vi "AFM_Lithography.vi"() -> ()   [LabVIEW 2019]
uses:
  subVIs/Global Variables.vi
  <vilib>/Analysis/Matrix/Datatypes/RealMatrix.ctl
  <vilib>/Analysis/Matrix/NI_Matrix.lvlib
  <userlib>/LevyLab/Relay Box/Typedefs/Resistor--enum.ctl
  <userlib>/LevyLab/Relay Box/Relay-Box.lvclass
  subVIs/AFM API/AFM_Driver_Manager/AFM_Driver_Manager.lvclass
  <vilib>/vision/Image Controls.llb/IMAQ Image.ctl
  <userlib>/LevyLab/Configuration/Configuration.lvclass
  Controls/Configuration.ctl
  Classes/Parse/ParseVectorFile/ParseVectorFile.lvclass
  <vilib>/JKI/JKI SMO/SMO/SMO.lvclass
  Classes/Settings/Setting Database/Setting Database.lvclass
  Classes/Settings/Setting Database/Typedefs/PrivateEvents--Setting Database.Refresh.ctl
  Classes/Parse/Dot/Dot.lvclass
  Classes/Settings/Dot Settings/Dot Settings.lvclass
  Classes/Settings/Path Settings/Path Settings.lvclass
  Classes/Tool/Tool Data/Tool Data/Tool Data.lvclass
  Classes/Settings/Setting Database/Typedefs/PublicEvents--Setting Database.PathsUpdated.ctl
  Classes/Settings/Rectangle Settings/Rectangle Settings.lvclass
  Classes/Settings/Setting Database/Typedefs/PublicEvents--Setting Database.RectanglesUpdated.ctl
  Classes/Settings/Funnel Settings/Funnel Settings.lvclass
  Classes/Settings/Setting Database/Typedefs/PublicEvents--Setting Database.FunnelsUpdated.ctl
  Classes/Settings/Setting Database/Typedefs/PublicEvents--Setting Database.DotsUpdated.ctl
  Classes/Parse/ParsePaths/Path.lvclass
  Classes/Parse/Rectangle/Rectangle.lvclass
  Classes/Parse/Image/SVGImage.lvclass
  Classes/Tool/Tool Data/Tool Data/Typedefs/PrivateEvents--Tool Data.Update Objects.ctl
  <vilib>/Platform/browser.llb/Open URL in Default Browser (string).vi
  Classes/Selector/Selector.lvclass
  <vilib>/Utility/miscctls.llb/LVPositionTypeDef.ctl
  Classes/Settings/ObjectSettings/ObjectSettings.lvclass
  C:/Program Files (x86)/National Instruments/LabVIEW 2019/vi.lib/JKI/JKI SMO/SMO/SMO.lvclass
  C:/Users/Albro/Documents/GitHub/AFM-Lithography/lvsrc/Classes/Settings/ObjectSettings/ObjectSettings.lvclass
  Classes/Tool/Tool Path/Tool Path.lvclass
  Classes/Tool/Tool Funnel/Tool Funnel.lvclass
  Classes/Tool/Tool Rectangle/Tool Rectangle.lvclass
  Classes/Tool/Tool Dot/Tool Dots.lvclass
panel:
  in  "Listbox":i32(listbox)
  out "version":string
  out "Ready?":bool
  out "Estimated Time":string
  in  "Run":bool
  in  "Refresh Button":bool
  in  "Done":bool
  in  "Help":bool
  in  "Abort":bool
  out "Render":T1(plugin-control)
  in  "Settings":T2(tab)
  out "Status":string
  in  "Background Image":path caption="Path"
  in  "Inkscape File (.svg)":path caption="Path"
  in  "Hide Labels?":bool
  in  "Patterns":i32(listbox) caption="Patterns (drag-and-drop reorder)"
  in  "AFM Type":u16(ring) caption="Ring" items=["Asylum"]
  in  "Save Render":bool caption="Save"
  in  "Autosave?":bool
  in  "Autosave Path":path caption="Path"
  in  "Create Overlay":bool
  out "Image Filename":string
  in  "Image Data Range":cluster{dbl, dbl}(slide)={100.0, 0.0} scale=0.0..100.0
  in  "Page":u32 caption="Numeric" max=3
  in  "MCLB":i32(listbox) caption="Multicolumn Listbox 2"
  # "AFM Lithography"
  # "Render"
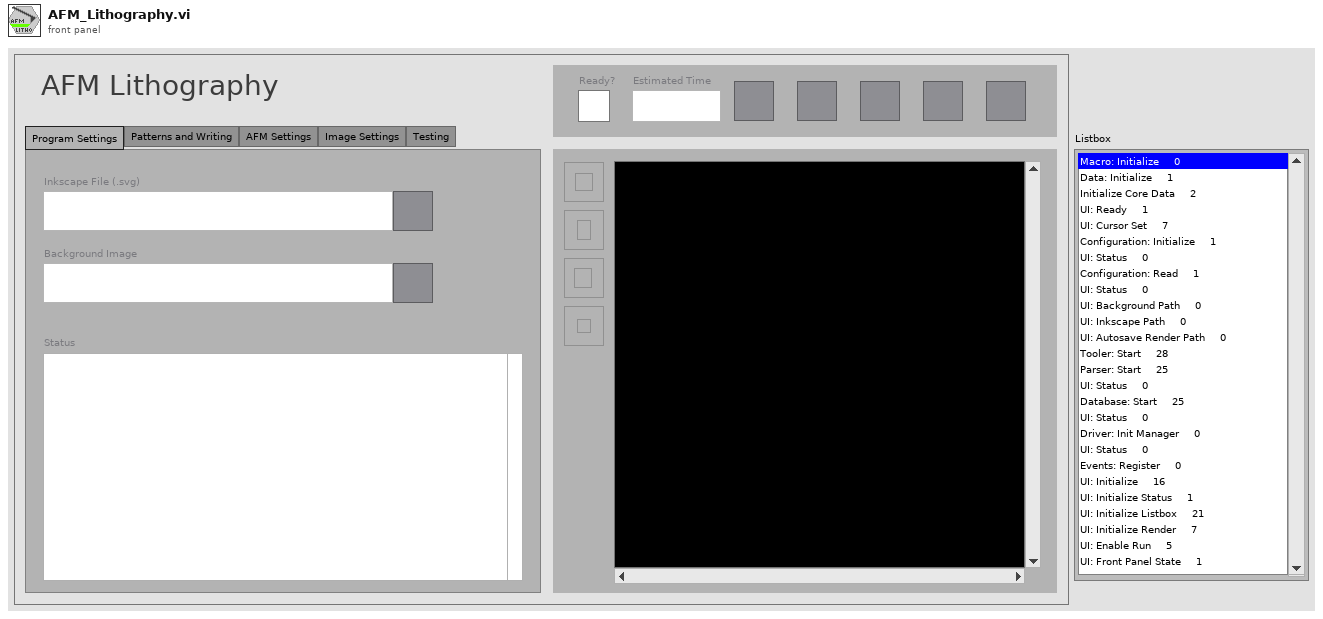
[diagram p1: front panel]
types:
  T1 = typedef "IMAQ Image.ctl" = refnum<image>
  T2 = enum32{"Program Settings", "Patterns and Writing", "AFM Settings", "Image Settings", "Testing"}
  T3 = typedef "LVPositionTypeDef.ctl" = cluster{"Left":i32, "Top":i32}
  T4 = cluster{"Point":T3, "Button":u16, "PlatMods":cluster{"Shift":bool, "Ctrl":bool, "Alt":bool, "Cmd":bool, "Opt":bool}}
  T5 = enum32{"invalid app kind", "Development System", "Run Time System", "Student Edition", "Embedded LabVIEW", "Evaluation", "Custom"}
  T6 = enum32{"Program Settings", "Patterns and Writing", "AFM Settings", "Image Settings"}
  T7 = enum32{"Invalid", "Standard", "Closed", "Hidden", "Minimized", "Maximized"}
  T8 = enum8{"Enabled", "Disabled", "Disabled and Grayed Out"}
  T9 = cluster{"Pattern":string, "Pattern Label":string, "Prompt":string}
  T10 = cluster{"Name":string, "Group":string, "Enabled":bool}
  T11 = typedef "Configuration.ctl" = cluster{"Inkscape Path":path, "Background Path":path, "Autosave Render Path":path, "Autosave Render":bool, "Hide Labels":bool, "Normal Render Path":path, "Overwrite":bool}
  T12 = typedef "Setting Database.lvclass/PrivateEvents--Setting Database.Refresh.ctl" = cluster{"Paths":string[], "Rectangles":string[], "Funnels":string[], "Dots":string[]}
  T13 = typedef "Tool Data.lvclass/PrivateEvents--Tool Data.Update Objects.ctl" = cluster{"Settings":cluster{"Paths":T14, "Rectangles":T15, "Funnels":T16, "Dots":T17}, "Data":cluster{"Paths":refnum<class "Path.lvclass">[], "Rectangles":refnum<class "Rectangle.lvclass">[], "SVGImage":refnum<class "SVGImage.lvclass">, "Dots":refnum<class "Dot.lvclass">[], "Funnels":refnum<class "Path.lvclass">[]}}
  T14 = typedef "Setting Database.lvclass/PublicEvents--Setting Database.PathsUpdated.ctl" = refnum<class "Path Settings.lvclass">[]
  T15 = typedef "Setting Database.lvclass/PublicEvents--Setting Database.RectanglesUpdated.ctl" = refnum<class "Rectangle Settings.lvclass">[]
  T16 = typedef "Setting Database.lvclass/PublicEvents--Setting Database.FunnelsUpdated.ctl" = refnum<class "Funnel Settings.lvclass">[]
  T17 = typedef "Setting Database.lvclass/PublicEvents--Setting Database.DotsUpdated.ctl" = refnum<class "Dot Settings.lvclass">[]
  T18 = typedef "NI_Matrix.lvlib/RealMatrix.ctl" = dbl[][]
  T19 = typedef "Relay-Box.lvclass/Resistor--enum.ctl" = enum16{"open", "discharge tip", "0 ohms", "100k ohm", "10M ohm", "1G ohm"}
  T20 = cluster{"Core":cluster{"Current VI Reference":refnum<vi>, "Close Panel on Exit?":bool}, "Parsing Data":cluster{"paths":cluster{"Fill Color":string, "Stroke Color":string, "Commands":cluster{"Command Type":string, "Coordinates":cluster{"X":dbl, "Y":dbl}[]}[], "Transformation Matrix 2":T18}[], "funnels":cluster{"Fill Color":string, "Stroke Color":string, "Commands":cluster{"Command Type":string, "Coordinates":cluster{"X":dbl, "Y":dbl}[]}[], "Transformation Matrix 2":T18}[], "rects":cluster{"Fill Color":string, "Stroke Color":string, "Width":dbl, "Height":dbl, "X":dbl, "Y":dbl, "Transformation Matrix":T18}[], "Dots":refnum<class "Dot.lvclass">[]}, "Lithography Data":cluster{"Name":string, "Litho":cluster{"X":dbl, "Y":dbl, "Speed":dbl, "Voltage":dbl}[], "Set Resistance":T19, "Meta":variant}[], "VI Refs":refnum<vi>[], "root path":path, "AFM_Driver_Manager":refnum<class "AFM_Driver_Manager.lvclass">, "IMAQ (Work)":T1, "Background Image":path, "Inkscape File (.svg)":path, "ParseVectorFile":refnum<class "ParseVectorFile.lvclass">, "Database":refnum<class "Setting Database.lvclass">, "Hide Labels":bool, "Autosave?":bool, "Autosave Path":path, "Image Data Range":cluster{dbl, dbl}, "Status":string, "Config":refnum<class "Configuration.lvclass">, "Drag and Drop":cluster{"Start":string[], "End":string[], "Running":string[], "Working":string[]}, "IDs":cluster{"paths":string[], "funnels":string[], "rects":string[], "dots":string[]}, "Tooler":refnum<class "Tool Data.lvclass">, "MCLB":refnum<class "Selector.lvclass">, "Menu Path":string, "Item Names":string[][]}
  T21 = cluster{"Paths":T14, "Rectangles":T15, "Funnels":T16, "Dots":T17}
  T22 = typedef "LVPoint32TypeDef.ctl" = cluster{"Horizontal":i32, "Vertical":i32}
  T23 = cluster{"Shift":bool, "Ctrl":bool, "Alt":bool, "Cmd":bool, "Opt":bool}
  T24 = cluster{"paths":string[], "funnels":string[], "rects":string[], "dots":string[]}
  T25 = cluster{"Start":string[], "End":string[], "Running":string[], "Working":string[]}
  T26 = cluster{"paths":cluster{"Fill Color":string, "Stroke Color":string, "Commands":cluster{"Command Type":string, "Coordinates":cluster{"X":dbl, "Y":dbl}[]}[], "Transformation Matrix 2":T18}[], "funnels":cluster{"Fill Color":string, "Stroke Color":string, "Commands":cluster{"Command Type":string, "Coordinates":cluster{"X":dbl, "Y":dbl}[]}[], "Transformation Matrix 2":T18}[], "rects":cluster{"Fill Color":string, "Stroke Color":string, "Width":dbl, "Height":dbl, "X":dbl, "Y":dbl, "Transformation Matrix":T18}[], "Dots":refnum<class "Dot.lvclass">[]}
  T27 = cluster{"Name":string, "Litho":cluster{"X":dbl, "Y":dbl, "Speed":dbl, "Voltage":dbl}[], "Set Resistance":T19, "Meta":variant}[]
  T28 = cluster{"Current VI Reference":refnum<vi>, "Close Panel on Exit?":bool}
  T29 = typedef "Setting Database.lvclass/PublicEvents--Cluster.ctl" = cluster{"NewActivePath":refnum<user-event>, "PathsUpdated":refnum<user-event>, "RectanglesUpdated":refnum<user-event>, "NewActiveRectangle":refnum<user-event>, "NewActiveFunnel":refnum<user-event>, "FunnelsUpdated":refnum<user-event>, "NewActiveDot":refnum<user-event>, "DotsUpdated":refnum<user-event>}
  T30 = typedef "AFM_Driver_Manager.lvclass/AFM_Driver_Manager.PublicEvents.ctl" = cluster{"Lithography Done":refnum<user-event>}
  T31 = typedef "Image Type" = u32
  T32 = cluster{"Name":string, "Litho":cluster{"X":dbl, "Y":dbl, "Speed":dbl, "Voltage":dbl}[], "Set Resistance":T19, "Meta":variant}
  T33 = cluster{"Name":string, "Group":string, "Enabled":bool}[]
  T34 = typedef "ParseVectorFile.lvclass/PublicEvents--ParseVectorFile.ParsedData.ctl" = cluster{"Paths":refnum<class "Path.lvclass">[], "Rectangles":refnum<class "Rectangle.lvclass">[], "Background":refnum<class "SVGImage.lvclass">, "Dots":refnum<class "Dot.lvclass">[], "Other Images":refnum<class "SVGImage.lvclass">[]}
  T35 = cluster{"Paths":refnum<class "Path.lvclass">[], "Rectangles":refnum<class "Rectangle.lvclass">[], "SVGImage":refnum<class "SVGImage.lvclass">, "Dots":refnum<class "Dot.lvclass">[], "Funnels":refnum<class "Path.lvclass">[]}
  T36 = typedef "Tool Data.lvclass/PublicEvents--Tool Data.Objects Updated.ctl" = cluster{"Paths":refnum<class "Tool Path.lvclass">[], "Funnels":refnum<class "Tool Funnel.lvclass">[], "Rectangles":refnum<class "Tool Rectangle.lvclass">[], "Dots":refnum<class "Tool Dots.lvclass">[]}
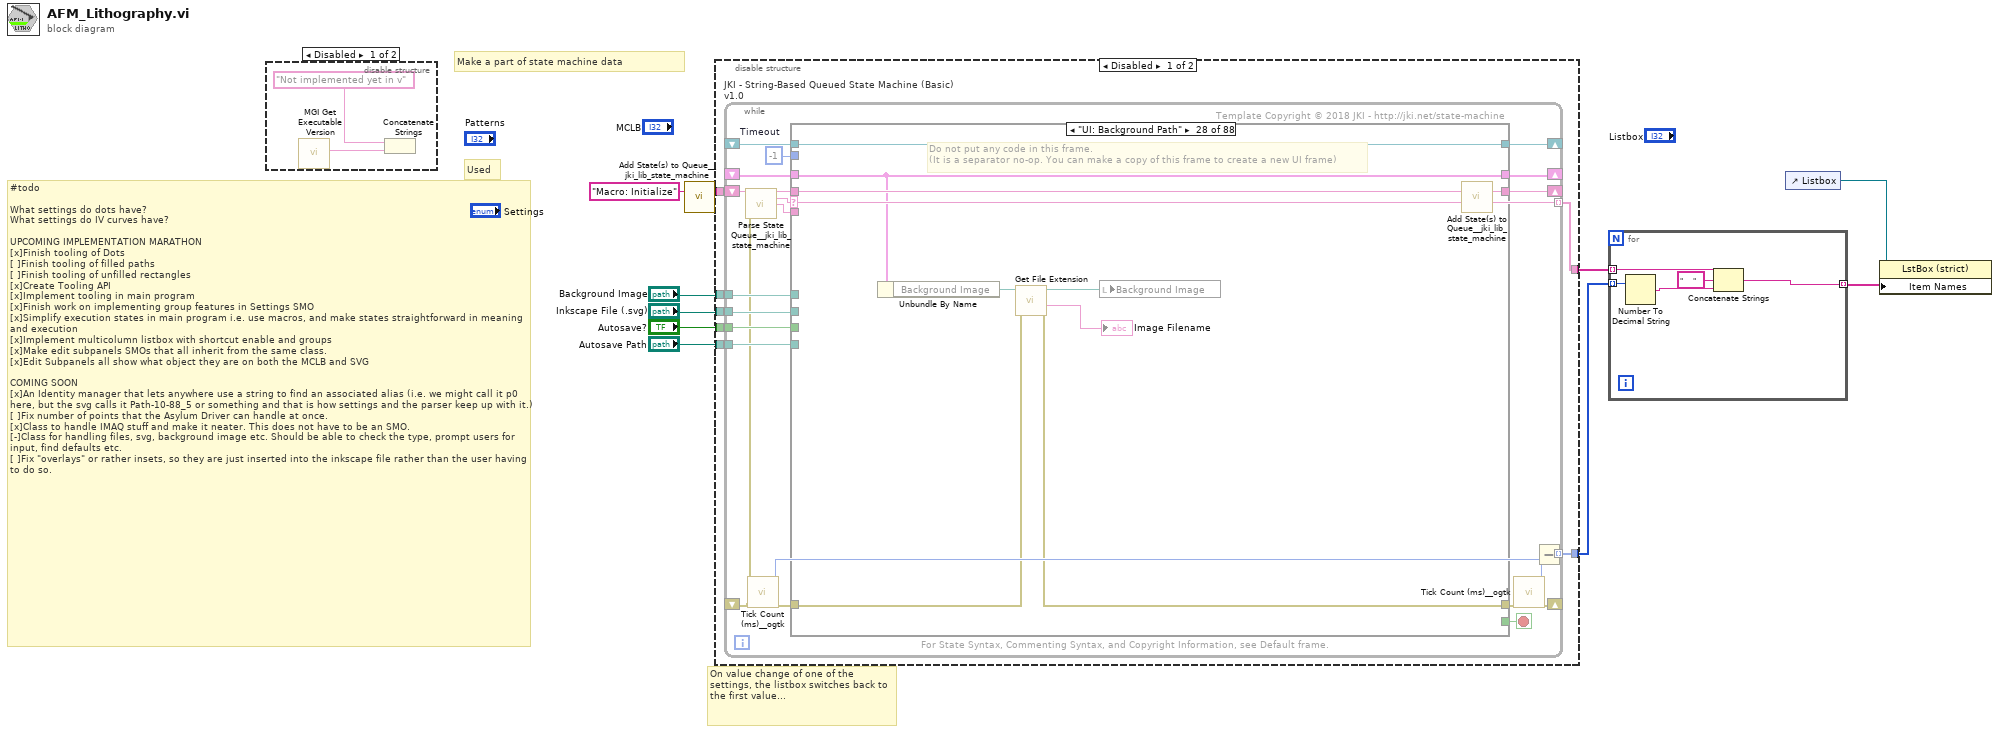
[diagram p0: block diagram]
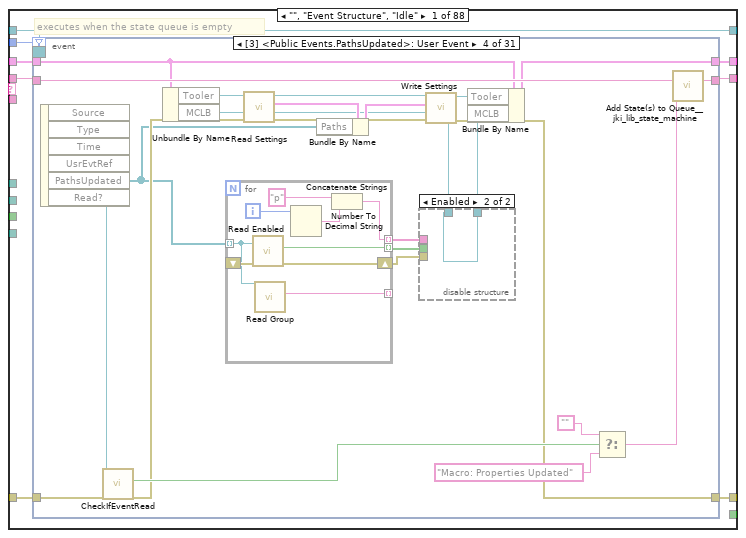
[diagram p2: hidden frame]
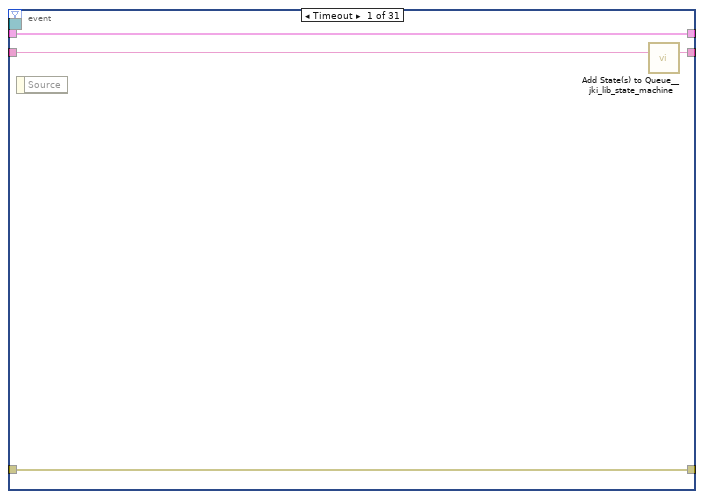
[diagram p3: hidden frame]
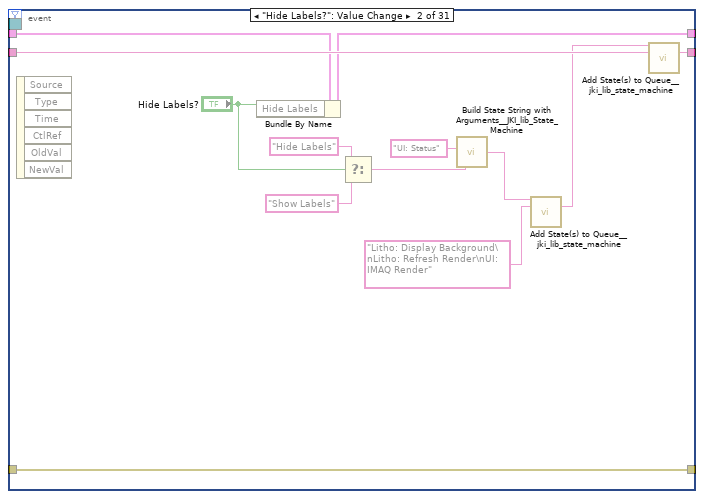
[diagram p4: hidden frame]
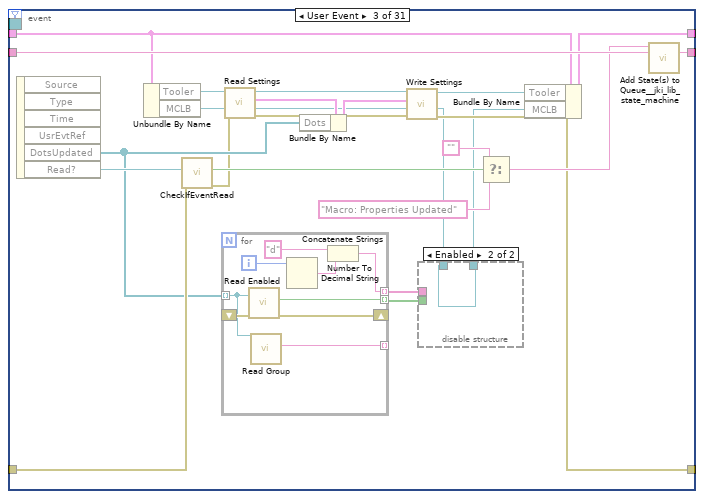
[diagram p5: hidden frame]
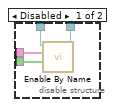
[diagram p6: hidden frame]
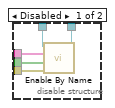
[diagram p7: hidden frame]
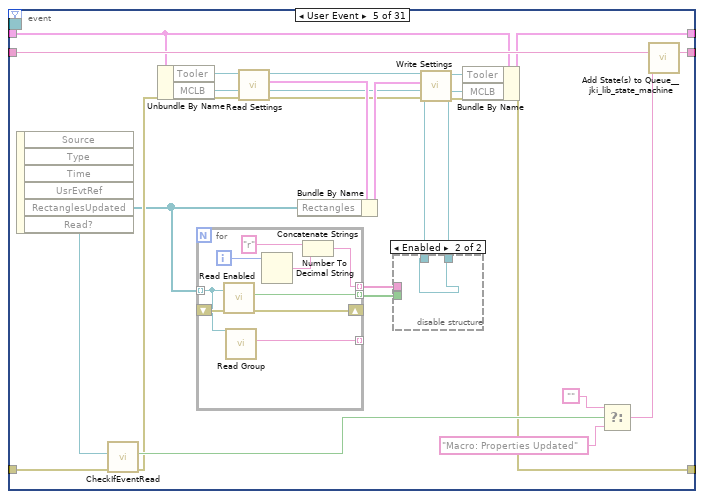
[diagram p8: hidden frame]
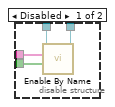
[diagram p9: hidden frame]
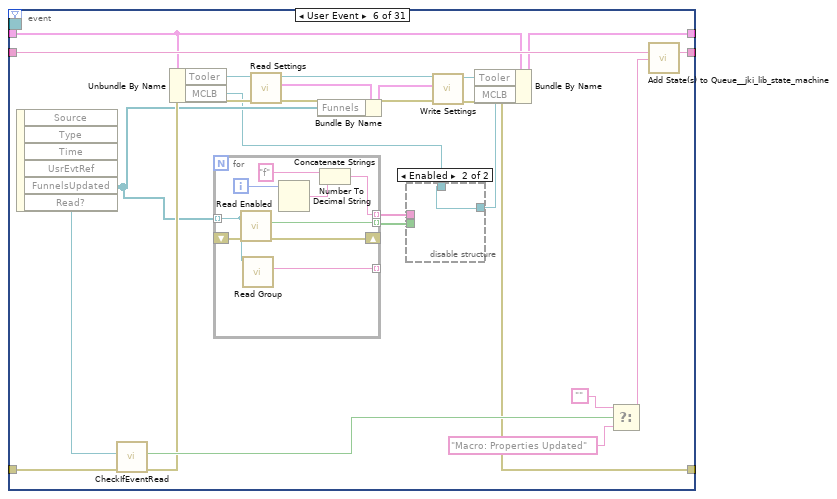
[diagram p10: hidden frame]
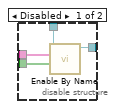
[diagram p11: hidden frame]
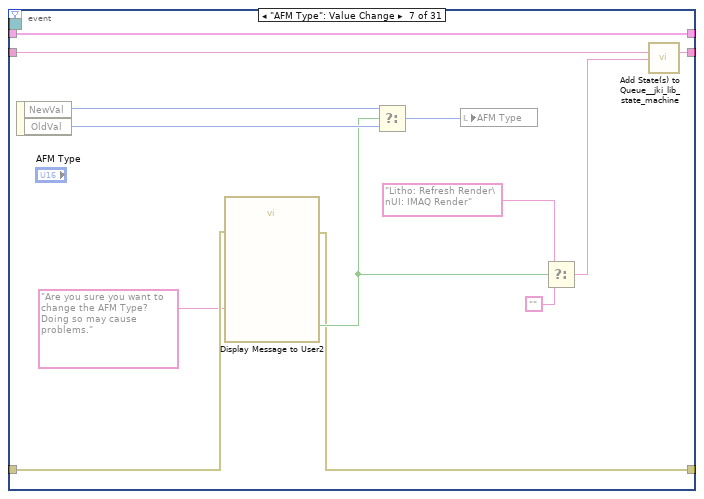
[diagram p12: hidden frame]
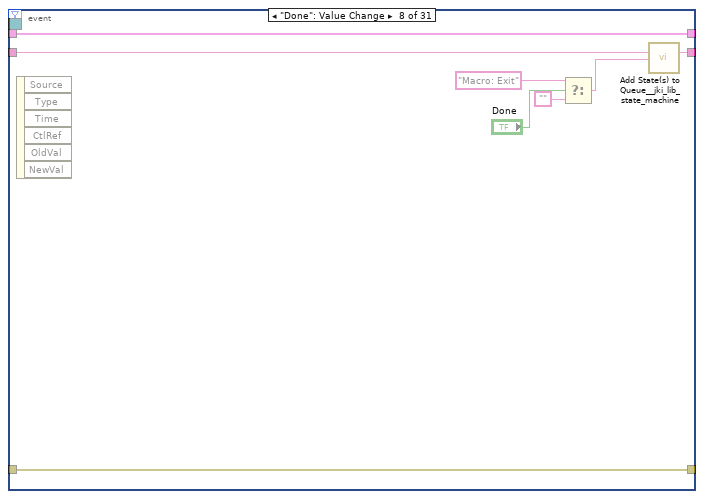
[diagram p13: hidden frame]
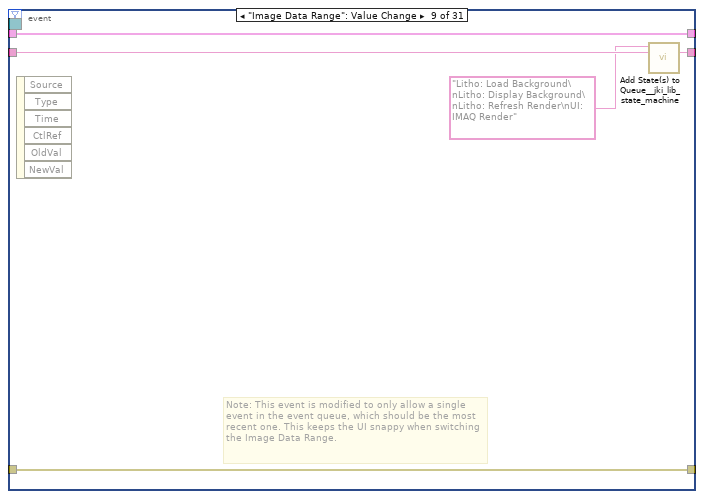
[diagram p14: hidden frame]
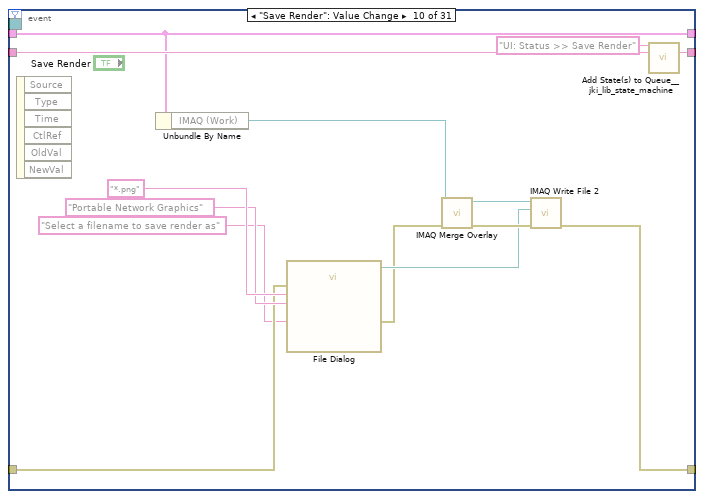
[diagram p15: hidden frame]
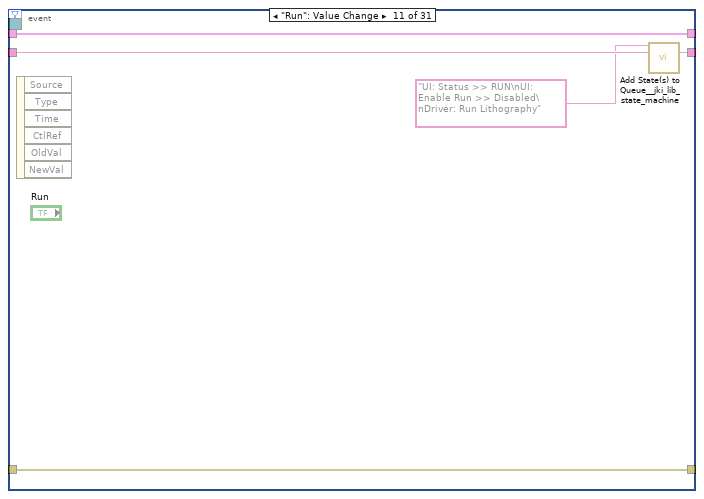
[diagram p16: hidden frame]
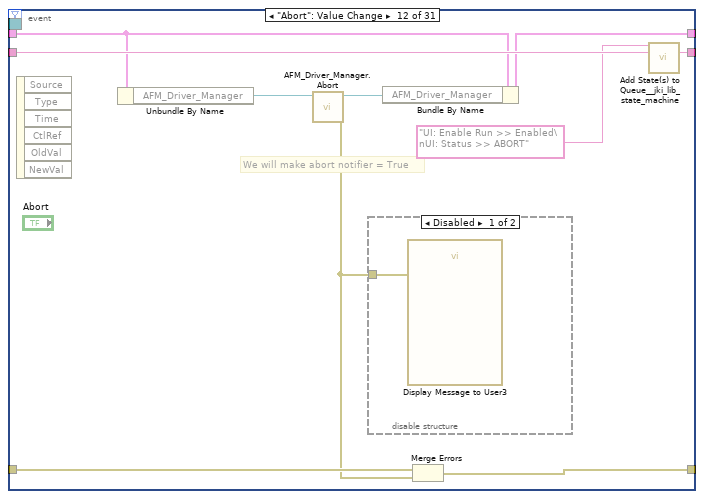
[diagram p17: hidden frame]
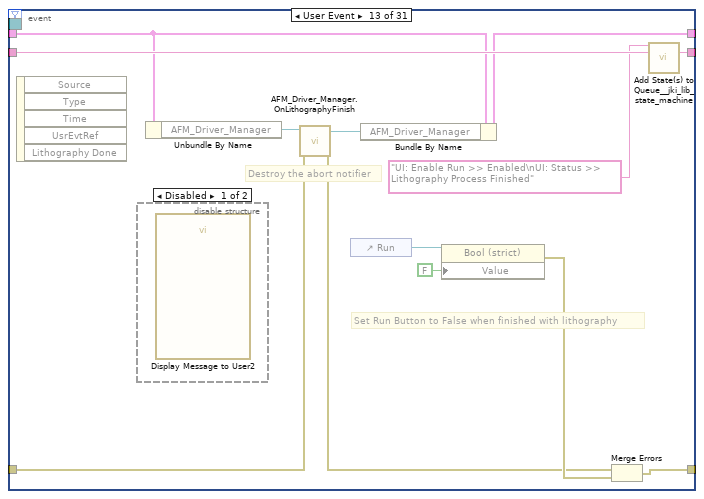
[diagram p19: hidden frame]
diagram:
  # "On value change of one of the settings, the listbox switches back to the first value..."
  # "#todo\n\nWhat settings do dots have?\nWhat settings do IV curves have?\n\nUPCOMING IMPLEMENTATION MARATHON\n[x]Finish tooling of Dots\n[ ]Finish tooling of filled paths\n[ ]Finish tooling of unfilled rectangles\n[x]Create Tooling API\n[x]Implement tooling in main program\n[x]Finish work on implementing group features in Settings SMO\n[x]Simplify execution states in main program i.e. use macros, and make states straightforward in meaning and execution\n[x]Implement multicolumn listbox with shortcut enable and groups\n[x]Make edit subpanels SMOs that all inherit from the same class.\n[x]Edit Subpanels all show what object they are on both the MCLB and SVG\n\nCOMING SOON\n[x]An Identity manager that lets anywhere use a string to find an associated alias (i.e. we might call it p0 here, but the svg calls it Path-10-88_5 or something and that is how settings and the parser keep up with it.)\n[ ]Fix number of points that the Asylum Driver can handle at once.\n[x]Class to handle IMAQ stuff and make it neater. This does not have to be an SMO.\n[-]Class for handling files, svg, background image etc. Should be able to check the type, prompt users for input, find defaults etc.\n[ ]Fix \"overlays\" or rather insets, so they are just inserted into the inkscape file rather than the user having to do so."
  # "Used"
  # "Make a part of state machine data"
  n1 = disable-structure shown="Disabled" {
    frame Disabled {
      n2 = call <userlib>:"MGI Get Executable Version.vi"() -> ("Version"=w11:string)  [unwired: 7 in]
      n3 = Concatenate Strings("Not implemented yet in v" ("Status"), w11) -> ()  [unwired: 1 out]
    }
    frame Enabled {
    }
  }
  n4 = call <vilib>:"Add State(s) to Queue__jki_lib_state_machine.vi"("State(s) in (\"\")"="Macro: Initialize") -> ("States Out"=w10:string)  [unwired: 14 in]
  n5 = disable-structure shown="Disabled" {
    disable-tunnel: w10 -> [w19 _]
    disable-tunnel: "Background Image" -> [w18 _]
    disable-tunnel: "Inkscape File (.svg)" -> [w17 _]
    disable-tunnel: "Autosave?" -> [w16 _]
    disable-tunnel: "Autosave Path" -> [w15 _]
    disable-tunnel: [w14 _] -> w4
    disable-tunnel: [w13 _] -> w3
    frame Disabled {
      n6 = while "JKI - String-Based Queued State Machine (Basic) v1.0" {
        shift-right: [w39] -> _
        shift-left: _ -> [w38]
        shift-right: [w24] -> _
        shift-left: _ -> [w26]
        shift-right: [w29] -> _
        shift-left: w19 -> [w41]
        shift-right: [w35] -> _
        shift-left: _ -> [w34]
        tunnel: w18 -> [w33]
        tunnel: w17 -> [w32]
        tunnel: w16 -> [w31]
        tunnel: w15 -> [w30]
        tunnel: [w25] -> w14 mode=indexing
        tunnel: [w20] -> w13 mode=indexing
        stop <- w40 stop-if-true
        w37 = -1  # Timeout
        # "Template Copyright © 2018 JKI - http://jki.net/state-machine"
        # "For State Syntax, Commenting Syntax, and Copyright Information, see Default frame."
        n7 = call <vilib>:"Parse State Queue__jki_lib_state_machine.vi"("State Queue"=w41, "Error In (no error)"=w26) -> ("Remaining States"=w36:string, "Current State"=w25:string, "Arguments"=w28:string)  [unwired: 11 in]
        n8 = call <userlib>:"Tick Count (ms)__ogtk.vi"("error in (no error)"=w26) -> ("error out"=w23:errorcluster, "millisecond timer value"=w21:u32)  [unwired: 9 in]
        n9 = case shown="\"UI: Background Path\"" w25 {
          selector: w25 -> [_ _ w478 _ _ _ _ _ _ _ _ _ _ _ _ _ _ _ _ _ _ _ _ _ _ _ _ _ _ _ _ _ _ _ _ _ _ _ _ _ _ _ _ _ _ _ _ _ _ _ _ _ _ _ _ _ _ _ _ _ _ _ _ _ _ _ _ _ _ _ _ _ _ _ _ _ _ _ _ _ _ _ _ _ _ _ _ _]
          tunnel: w28 -> [_ _ _ _ w505 _ _ _ _ _ _ _ _ _ _ _ _ _ _ w688 w700 w708 w724 w735 _ w778 _ _ _ _ _ _ _ _ _ _ _ _ _ _ _ _ _ _ _ _ _ _ _ _ _ _ _ _ _ _ _ _ _ _ _ _ _ _ _ _ _ w1320 _ _ _ _ _ _ _ _ _ _ w1452 w1462 _ _ _ _ _ _ _ _]
          tunnel: w38 -> [w46 w473 w480 w494 w503 w512 w517 _ w554 w573 w586 w595 w602 w615 w619 w637 w645 w652 w680 w694 w704 w710 w714 w733 w764 w781 w785 w795 w812 w821 w830 w855 w875 w879 w885 w891 w896 w902 w908 w914 w920 w930 w935 w945 w964 w989 w1018 w1028 w1037 w1073 w1083 w1094 w1125 w1133 w1156 w1164 w1178 w1192 w1198 w1221 w1237 w1254 w1272 w1284 w1291 w1295 w1306 w1325 w1336 w1344 w1354 w1364 w1378 w1382 w1415 w1428 w1440 w1446 w1457 w1470 w1517 w1556 w1571 w1583 w1590 w1601 w1612 w1642]
          tunnel: w23 -> [w49 w476 w486 w501 w509 w515 w520 w523 w559 w577 w579 w598 w604 w613 w622 w628 w640 w648 w672 w698 w707 w713 w715 w739 w765 w772 w789 w792 w808 w817 w829 w834 w870 w882 w888 w894 w899 w905 w911 w917 w923 w932 w943 w948 w962 w987 w1021 w1030 w1034 w1063 w1085 w1101 w1120 w1141 w1161 w1163 w1183 w1189 w1203 w1226 w1242 w1246 w1269 w1280 w1293 w1296 w1314 w1322 w1333 w1346 w1351 w1368 w1375 w1387 w1391 w1423 w1434 w1451 w1453 w1467 w1508 w1543 w1562 w1577 w1589 w1595 w1606 w1631]
          tunnel: [w47 w475 w482 w500 w507 w514 w519 w549 w555 w576 w589 w597 w611 w617 w621 w635 w647 w668 w678 w697 w706 w712 w725 w737 w769 w783 w788 w798 w815 w826 w833 w856 w877 w881 w887 w893 w898 w904 w910 w916 w922 w931 w942 w947 w967 w993 w1024 w1029 w1039 w1080 w1084 w1100 w1128 w1140 w1160 w1168 w1182 w1196 w1202 w1225 w1241 w1258 w1276 w1288 w1292 w1303 w1317 w1329 w1340 w1350 w1361 w1372 w1380 w1386 w1420 w1432 w1444 w1450 w1461 w1474 w1521 w1560 w1575 w1587 w1594 w1605 w1616 w1646] -> w29
          tunnel: [_ _ _ _ _ TRUE _ _ _ _ _ _ _ _ _ _ _ _ _ _ _ _ _ _ _ _ _ _ _ _ _ _ _ _ _ _ _ _ _ _ _ _ _ _ _ _ _ _ _ _ _ _ _ _ _ _ _ _ _ _ _ _ _ _ _ _ _ _ _ _ _ _ _ _ _ _ _ _ _ _ _ _ _ _ _ _ _ _] -> w40
          tunnel: [w45 w473 w480 w493 w503 w512 w517 w547 w557 w574 w586 w595 w602 w615 w619 w637 w645 w650 w680 w693 w704 w710 w714 w733 w764 w781 w785 w795 w812 w821 w830 w855 w875 w879 w885 w891 w896 w902 w908 w914 w920 w930 w935 w945 w963 w990 w1022 w1028 w1038 w1074 w1083 w1093 w1125 w1134 w1157 w1165 w1179 w1193 w1199 w1222 w1238 w1255 w1273 w1285 w1291 w1299 w1313 w1327 w1337 w1345 w1356 w1367 w1378 w1383 w1416 w1429 w1441 w1447 w1458 w1471 w1518 w1557 w1572 w1584 w1591 w1602 w1613 w1643] -> w39
          tunnel: w37 -> [w44 _ _ _ _ _ _ _ _ _ _ _ _ _ _ _ _ _ _ _ _ _ _ _ _ _ _ _ _ _ _ _ _ _ _ _ _ _ _ _ _ _ _ _ _ _ _ _ _ _ _ _ _ _ _ _ _ _ _ _ _ _ _ _ _ _ _ _ _ _ _ _ _ _ _ _ _ _ _ _ _ _ _ _ _ _ _ _]
          tunnel: [w48 w476 w487 w501 errorcluster {"status"=FALSE, "code"=0, "source"=""} ("error out") w515 w520 w524 w558 w577 w590 w598 w605 w612 w622 w631 w641 w656 w673 w698 w707 w713 w719 w738 w766 w773 w789 w793 w801 w818 w829 w836 w869 w882 w888 w894 w899 w905 w911 w917 w923 w932 w943 w948 w958 w982 w1014 w1030 w1033 w1062 w1085 w1101 w1119 w1141 w1161 w1163 w1183 w1189 w1203 w1226 w1242 w1245 w1264 w1281 w1293 w1297 w1315 w1323 w1334 w1347 w1352 w1369 w1376 w1387 w1400 w1424 w1435 w1451 w1454 w1468 w1506 w1522 w1564 w1578 w1589 w1596 w1607 w1629] -> w27
          tunnel: w36 -> [w43 w474 w481 w495 w504 w511 w518 w548 w555 w575 w585 w596 w610 w616 w620 w636 w646 w669 w679 w696 w705 w711 w723 w734 w768 w782 w787 w797 w814 w825 w832 w854 w876 w880 w886 w892 w897 w903 w909 w915 w921 w929 w934 w946 w966 w992 w1023 w1027 w1031 w1078 w1082 w1099 w1127 w1139 w1159 w1167 w1181 w1195 w1201 w1224 w1240 w1257 w1275 w1287 w1290 w1302 w1316 w1328 w1339 w1349 w1360 w1371 w1379 w1385 w1419 w1431 w1443 w1449 w1460 w1473 w1520 w1559 w1574 w1586 w1593 w1604 w1615 w1645]
          tunnel: [w42 w472 w477 w489 w502 w510 w516 w546 w551 w570 w582 w594 w609 w614 w618 w634 w644 w659 w674 w695 w703 w709 w722 w732 w767 w780 w786 w796 w813 w824 w831 w853 w871 w878 w884 w889 w895 w901 w907 w913 w919 w925 w933 w944 w965 w991 w1013 w1026 w1036 w1077 w1081 w1098 w1126 w1138 w1158 w1166 w1180 w1194 w1200 w1223 w1239 w1256 w1274 w1286 w1289 w1301 w1308 w1321 w1331 w1342 w1355 w1365 w1374 w1384 w1418 w1430 w1442 w1448 w1459 w1472 w1519 w1558 w1573 w1585 w1592 w1603 w1614 w1644] -> w35
          tunnel: w34 -> [w42 w472 w477 w489 w502 w510 w516 w546 w551 w570 w582 w594 _ w614 w618 w634 w644 w659 w674 w695 w703 w709 w722 w732 w767 w780 w786 w796 w813 w824 w831 w853 w871 w878 w884 w889 w895 w901 w907 w913 w919 w925 w933 w944 w965 w991 w1013 w1026 w1036 w1077 w1081 w1098 w1126 w1138 w1158 w1166 w1180 w1194 w1200 w1223 w1239 w1256 w1274 w1286 w1289 w1301 w1308 w1321 w1331 w1342 w1355 w1365 w1374 w1384 w1418 w1430 w1442 w1448 w1459 w1472 w1519 w1558 w1573 w1585 w1592 w1603 w1614 w1644]
          tunnel: w33 -> [_ _ _ _ _ _ _ w545 _ _ _ _ _ _ _ _ _ _ _ _ _ _ _ _ _ _ _ _ _ _ _ _ _ _ _ _ _ _ _ _ _ _ _ _ _ _ _ _ _ _ _ _ _ _ _ _ _ _ _ _ _ _ _ _ _ _ _ _ _ _ _ _ _ _ _ _ _ _ _ _ _ _ _ _ _ _ _ _]
          tunnel: w32 -> [_ _ _ _ _ _ _ w544 _ _ _ _ _ _ _ _ _ _ _ _ _ _ _ _ _ _ _ _ _ _ _ _ _ _ _ _ _ _ _ _ _ _ _ _ _ _ _ _ _ _ _ _ _ _ _ _ _ _ _ _ _ _ _ _ _ _ _ _ _ _ _ _ _ _ _ _ _ _ _ _ _ _ _ _ _ _ _ _]
          tunnel: w31 -> [_ _ _ _ _ _ _ w534 _ _ _ _ _ _ _ _ _ _ _ _ _ _ _ _ _ _ _ _ _ _ _ _ _ _ _ _ _ _ _ _ _ _ _ _ _ _ _ _ _ _ _ _ _ _ _ _ _ _ _ _ _ _ _ _ _ _ _ _ _ _ _ _ _ _ _ _ _ _ _ _ _ _ _ _ _ _ _ _]
          tunnel: w30 -> [_ _ _ _ _ _ _ w533 _ _ _ _ _ _ _ _ _ _ _ _ _ _ _ _ _ _ _ _ _ _ _ _ _ _ _ _ _ _ _ _ _ _ _ _ _ _ _ _ _ _ _ _ _ _ _ _ _ _ _ _ _ _ _ _ _ _ _ _ _ _ _ _ _ _ _ _ _ _ _ _ _ _ _ _ _ _ _ _]
          frame "", "Event Structure", "Idle" {
            # "executes when the state queue is empty"
            n10 = event shown="[3] <Public Events.PathsUpdated>: User Event" {
              selector: w42 -> [_ _ _ _ _ _ _ _ _ _ _ _ _ _ _ _ _ _ _ _ _ _ _ _ _ _ _ _ _ _ _]
              dyn-events: _ -> [_ _ _ _ _ _ _ _ _ _ _ _ _ _ _ _ _ _ _ _ _ _ _ _ _ _ _ _ _ _ _]
              timeout: w44 -> [_ _ _ _ _ _ _ _ _ _ _ _ _ _ _ _ _ _ _ _ _ _ _ _ _ _ _ _ _ _ _]
              tunnel: w43 -> [w53 w66 w89 w127 w165 w202 w227 w234 w239 w255 w258 w270 w284 w287 w302 w313 w325 w332 w337 w342 w347 w351 w362 w373 w390 w408 w439 w443 w453 w464 w470]
              tunnel: [w52 w65 w88 w126 w164 w201 w228 w235 w240 w256 w259 w271 w285 w288 w301 w312 w324 w331 w336 w341 w346 w350 w361 w372 w389 w407 w438 w442 w452 w463 w469] -> w47
              tunnel: w46 -> [w51 w62 w73 w113 w151 w188 w229 w236 w241 w254 w260 w265 w277 w290 w299 w310 w323 w328 w334 w340 w348 w352 w358 w368 w387 w403 w435 w444 w449 w460 w468]
              tunnel: w49 -> [w50 w64 w83 w125 w161 w198 w219 w237 w242 w246 w261 w267 w278 w292 w303 w314 w326 w333 w338 w343 w344 w353 w354 w364 w391 w397 w440 w445 w447 w465 w471]
              tunnel: [w51 w63 w78 w111 w148 w185 w229 w236 w241 w254 w260 w266 w280 w290 w300 w311 w316 w329 w334 w340 w348 w352 w359 w369 w388 w402 w436 w444 w450 w461 w468] -> w45
              tunnel: [w50 w64 w74 w105 w149 w186 w218 w237 w242 w250 w261 w268 w274 w291 w303 w314 w326 w333 w338 w343 w344 w353 w355 w365 w391 w398 w440 w445 w446 w465 w471] -> w48
              event Timeout {
                n11 = event-data() -> ()  [unwired: 1 in, 1 out]
                n12 = call <vilib>:"Add State(s) to Queue__jki_lib_state_machine.vi"("State(s) in (\"\")"=w53) -> ("States Out"=w52:string)  [unwired: 14 in]
              }
              event "Hide Labels?": Value Change {
                n13 = event-data() -> ()  [unwired: 1 in, 6 out]
                n14 = Bundle By Name(cluster=w62, "Hide Labels"="Hide Labels?") -> (w63:T20)
                n15 = Select(t="Hide Labels" ("State(s) in Front (\"\")"), s="Hide Labels?", f="Show Labels" ("State(s) in Front (\"\")")) -> (s? t:f=w57:string)
                n16 = call <vilib>:"Build State String with Arguments__JKI_lib_State_Machine.vi"("Arguments (\"\")"=w57, "State"="UI: Status") -> ("State with Arguments"=w56:string)  [unwired: 4 in]
                n17 = call <vilib>:"Add State(s) to Queue__jki_lib_state_machine.vi"("State(s) in Front (\"\")"=w56, "State(s) in (\"\")"="Litho: Display Background\nLitho: Refresh Render\nUI: IMAQ Render") -> ("States Out"=w60:string)  [unwired: 13 in]
                n18 = call <vilib>:"Add State(s) to Queue__jki_lib_state_machine.vi"("State(s) in Front (\"\")"=w60, "State(s) in (\"\")"=w66) -> ("States Out"=w65:string)  [unwired: 13 in]
              }
              event User Event {
                n19 = event-data() -> ("DotsUpdated"=w72:T17, "Read?"=w87:refnum<notifier>)  [unwired: 1 in, 4 out]
                n20 = Unbundle By Name(w73) -> ("Tooler"=w81:refnum<class "Tool Data.lvclass">, "MCLB"=w69:refnum<class "Selector.lvclass">)
                n21 = call "CheckIfEventRead.vi"("error in (no error)"=w83, "Read?"=w87) -> ("error out"=w67:errorcluster, "Read"=w82:bool)  [unwired: 8 in]
                n22 = for {
                  tunnel: w72 -> [w96] mode=indexing
                  tunnel: [w103] -> w70 mode=indexing
                  tunnel: [w99] -> w71 mode=indexing
                  shift-right: [w98] -> _
                  shift-left: _ -> [w97]
                  tunnel: [w95] -> _ mode=indexing
                  i -> [w101]
                  n23 = call "Read Enabled.vi"("error in (no error)"=w97, "ObjectSettings in"=w96) -> ("error out"=w98:errorcluster, "Enabled"=w103:bool)  [unwired: 7 in, 1 out]
                  n24 = call-dynamic "Read Group.vi"("ObjectSettings in"=w96) -> ("Group"=w95:string)  [unwired: 8 in, 2 out]
                  n25 = Number To Decimal String(number=w101) -> (decimal integer string=w100:string)  [unwired: 1 in]
                  n26 = Concatenate Strings("d" ("string"), w100) -> (w99:string)
                }
                n27 = call-dynamic "Read Settings.vi"("error in (no error)"=w67, "Tool Data in"=w81) -> ("error out"=w75:errorcluster, "Settings"=w77:T21, "Tool Data out"=w80:refnum<class "Tool Data.lvclass">)  [unwired: 7 in]
                n28 = Bundle By Name(cluster=w77, "Dots"=w72) -> (w76:T21)
                n29 = call-dynamic "Write Settings.vi"("error in (no error)"=w75, "Settings"=w76, "Tool Data in"=w80) -> ("error out"=w74:errorcluster, "Tool Data out"=w79:refnum<class "Tool Data.lvclass">)  [unwired: 7 in]
                n30 = disable-structure shown="Enabled" {
                  disable-tunnel: w71 -> [w93 _]
                  disable-tunnel: w70 -> [w92 _]
                  disable-tunnel: w69 -> [w91 w94]
                  disable-tunnel: [w90 w94] -> w68
                  frame Disabled {
                    n31 = call-dynamic "Enable By Name.vi"("Enable Items"=w92, "Names"=w93, "Selector in"=w91) -> ("Selector out"=w90:refnum<class "Selector.lvclass">)  [unwired: 7 in, 1 out]
                  }
                  frame Enabled {
                  }
                }
                n32 = Select(t="", s=w82, f="Macro: Properties Updated") -> (s? t:f=w84:string)
                n33 = Bundle By Name(cluster=w73, "Tooler"=w79, "MCLB"=w68) -> (w78:T20)
                n34 = call <vilib>:"Add State(s) to Queue__jki_lib_state_machine.vi"("State(s) in Front (\"\")"=w84, "State(s) in (\"\")"=w89) -> ("States Out"=w88:string)  [unwired: 13 in]
              }
              event User Event {
                n35 = event-data() -> ("PathsUpdated"=w108:T14, "Read?"=w124:refnum<notifier>)  [unwired: 1 in, 4 out]
                n36 = call "CheckIfEventRead.vi"("error in (no error)"=w125, "Read?"=w124) -> ("error out"=w112:errorcluster, "Read"=w120:bool)  [unwired: 8 in]
                n37 = Unbundle By Name(w113) -> ("Tooler"=w119:refnum<class "Tool Data.lvclass">, "MCLB"=w107:refnum<class "Selector.lvclass">)
                n38 = for {
                  tunnel: w108 -> [w135] mode=indexing
                  tunnel: [w142] -> w109 mode=indexing
                  tunnel: [w138] -> w110 mode=indexing
                  shift-right: [w137] -> w104
                  shift-left: _ -> [w136]
                  tunnel: [w134] -> _ mode=indexing
                  i -> [w140]
                  n39 = call "Read Enabled.vi"("error in (no error)"=w136, "ObjectSettings in"=w135) -> ("error out"=w137:errorcluster, "Enabled"=w142:bool)  [unwired: 7 in, 1 out]
                  n40 = call-dynamic "Read Group.vi"("ObjectSettings in"=w135) -> ("Group"=w134:string)  [unwired: 8 in, 2 out]
                  n41 = Number To Decimal String(number=w140) -> (decimal integer string=w139:string)  [unwired: 1 in]
                  n42 = Concatenate Strings("p" ("string"), w139) -> (w138:string)
                }
                n43 = call-dynamic "Read Settings.vi"("error in (no error)"=w112, "Tool Data in"=w119) -> ("error out"=w114:errorcluster, "Settings"=w116:T21, "Tool Data out"=w118:refnum<class "Tool Data.lvclass">)  [unwired: 7 in]
                n44 = Bundle By Name(cluster=w116, "Paths"=w108) -> (w115:T21)
                n45 = disable-structure shown="Enabled" {
                  disable-tunnel: w110 -> [w132 _]
                  disable-tunnel: w109 -> [w131 _]
                  disable-tunnel: w107 -> [w130 w133]
                  disable-tunnel: [w129 w133] -> w106
                  disable-tunnel: w104 -> [w128 _]
                  frame Disabled {
                    n46 = call-dynamic "Enable By Name.vi"("error in (no error)"=w128, "Enable Items"=w131, "Names"=w132, "Selector in"=w130) -> ("Selector out"=w129:refnum<class "Selector.lvclass">)  [unwired: 6 in, 1 out]
                  }
                  frame Enabled {
                  }
                }
                n47 = call-dynamic "Write Settings.vi"("error in (no error)"=w114, "Settings"=w115, "Tool Data in"=w118) -> ("error out"=w105:errorcluster, "Tool Data out"=w117:refnum<class "Tool Data.lvclass">)  [unwired: 7 in]
                n48 = Bundle By Name(cluster=w113, "Tooler"=w117, "MCLB"=w106) -> (w111:T20)
                n49 = Select(t="", s=w120, f="Macro: Properties Updated") -> (s? t:f=w121:string)
                n50 = call <vilib>:"Add State(s) to Queue__jki_lib_state_machine.vi"("State(s) in (\"\")"=w127, "State(s) at Back (\"\")"=w121) -> ("States Out"=w126:string)  [unwired: 13 in]
              }
              event User Event {
                n51 = event-data() -> ("RectanglesUpdated"=w145:T15, "Read?"=w160:refnum<notifier>)  [unwired: 1 in, 4 out]
                n52 = call "CheckIfEventRead.vi"("error in (no error)"=w161, "Read?"=w160) -> ("error out"=w150:errorcluster, "Read"=w158:bool)  [unwired: 8 in]
                n53 = Unbundle By Name(w151) -> ("Tooler"=w157:refnum<class "Tool Data.lvclass">, "MCLB"=w144:refnum<class "Selector.lvclass">)
                n54 = for {
                  tunnel: w145 -> [w172] mode=indexing
                  tunnel: [w179] -> w146 mode=indexing
                  tunnel: [w175] -> w147 mode=indexing
                  shift-right: [w174] -> _
                  shift-left: _ -> [w173]
                  tunnel: [w171] -> _ mode=indexing
                  i -> [w177]
                  n55 = call "Read Enabled.vi"("error in (no error)"=w173, "ObjectSettings in"=w172) -> ("error out"=w174:errorcluster, "Enabled"=w179:bool)  [unwired: 7 in, 1 out]
                  n56 = call-dynamic "Read Group.vi"("ObjectSettings in"=w172) -> ("Group"=w171:string)  [unwired: 8 in, 2 out]
                  n57 = Number To Decimal String(number=w177) -> (decimal integer string=w176:string)  [unwired: 1 in]
                  n58 = Concatenate Strings("r" ("string"), w176) -> (w175:string)
                }
                n59 = call-dynamic "Read Settings.vi"("error in (no error)"=w150, "Tool Data in"=w157) -> ("error out"=w152:errorcluster, "Settings"=w154:T21, "Tool Data out"=w156:refnum<class "Tool Data.lvclass">)  [unwired: 7 in]
                n60 = Bundle By Name(cluster=w154, "Rectangles"=w145) -> (w153:T21)
                n61 = disable-structure shown="Enabled" {
                  disable-tunnel: w147 -> [w169 _]
                  disable-tunnel: w146 -> [w168 _]
                  disable-tunnel: w144 -> [w167 w170]
                  disable-tunnel: [w166 w170] -> w143
                  frame Disabled {
                    n62 = call-dynamic "Enable By Name.vi"("Enable Items"=w168, "Names"=w169, "Selector in"=w167) -> ("Selector out"=w166:refnum<class "Selector.lvclass">)  [unwired: 7 in, 1 out]
                  }
                  frame Enabled {
                  }
                }
                n63 = call-dynamic "Write Settings.vi"("error in (no error)"=w152, "Settings"=w153, "Tool Data in"=w156) -> ("error out"=w149:errorcluster, "Tool Data out"=w155:refnum<class "Tool Data.lvclass">)  [unwired: 7 in]
                n64 = Bundle By Name(cluster=w151, "Tooler"=w155, "MCLB"=w143) -> (w148:T20)
                n65 = Select(t="", s=w158, f="Macro: Properties Updated") -> (s? t:f=w159:string)
                n66 = call <vilib>:"Add State(s) to Queue__jki_lib_state_machine.vi"("State(s) in (\"\")"=w165, "State(s) at Back (\"\")"=w159) -> ("States Out"=w164:string)  [unwired: 13 in]
              }
              event User Event {
                n67 = event-data() -> ("FunnelsUpdated"=w182:T16, "Read?"=w197:refnum<notifier>)  [unwired: 1 in, 4 out]
                n68 = call "CheckIfEventRead.vi"("error in (no error)"=w198, "Read?"=w197) -> ("error out"=w187:errorcluster, "Read"=w195:bool)  [unwired: 8 in]
                n69 = Unbundle By Name(w188) -> ("Tooler"=w194:refnum<class "Tool Data.lvclass">, "MCLB"=w180:refnum<class "Selector.lvclass">)
                n70 = for {
                  tunnel: [w208] -> _ mode=indexing
                  tunnel: [w216] -> w183 mode=indexing
                  tunnel: [w212] -> w184 mode=indexing
                  shift-right: [w211] -> _
                  shift-left: _ -> [w210]
                  tunnel: [w209] -> _ mode=indexing
                  tunnel: w182 -> [w208] mode=indexing
                  i -> [w214]
                  n71 = call "Read Enabled.vi"("error in (no error)"=w210, "ObjectSettings in"=w208) -> ("error out"=w211:errorcluster, "Enabled"=w216:bool)  [unwired: 7 in, 1 out]
                  n72 = call-dynamic "Read Group.vi"("ObjectSettings in"=w208) -> ("Group"=w209:string)  [unwired: 8 in, 2 out]
                  n73 = Number To Decimal String(number=w214) -> (decimal integer string=w213:string)  [unwired: 1 in]
                  n74 = Concatenate Strings("f" ("string"), w213) -> (w212:string)
                }
                n75 = call-dynamic "Read Settings.vi"("error in (no error)"=w187, "Tool Data in"=w194) -> ("error out"=w189:errorcluster, "Settings"=w191:T21, "Tool Data out"=w193:refnum<class "Tool Data.lvclass">)  [unwired: 7 in]
                n76 = Bundle By Name(cluster=w191, "Funnels"=w182) -> (w190:T21)
                n77 = disable-structure shown="Enabled" {
                  disable-tunnel: w184 -> [w206 _]
                  disable-tunnel: w183 -> [w205 _]
                  disable-tunnel: [w204 w207] -> w181
                  disable-tunnel: w180 -> [w203 w207]
                  frame Disabled {
                    n78 = call-dynamic "Enable By Name.vi"("Enable Items"=w205, "Names"=w206, "Selector in"=w203) -> ("Selector out"=w204:refnum<class "Selector.lvclass">)  [unwired: 7 in, 1 out]
                  }
                  frame Enabled {
                  }
                }
                n79 = call-dynamic "Write Settings.vi"("error in (no error)"=w189, "Settings"=w190, "Tool Data in"=w193) -> ("error out"=w186:errorcluster, "Tool Data out"=w192:refnum<class "Tool Data.lvclass">)  [unwired: 7 in]
                n80 = Bundle By Name(cluster=w188, "Tooler"=w192, "MCLB"=w181) -> (w185:T20)
                n81 = Select(t="", s=w195, f="Macro: Properties Updated") -> (s? t:f=w196:string)
                n82 = call <vilib>:"Add State(s) to Queue__jki_lib_state_machine.vi"("State(s) in (\"\")"=w202, "State(s) at Back (\"\")"=w196) -> ("States Out"=w201:string)  [unwired: 13 in]
              }
              event "AFM Type": Value Change {
                n83 = event-data() -> ("NewVal"=w223:u16, "OldVal"=w222:u16)  [unwired: 1 in]
                n84 = call "Display Message to User2"("error in (no error)"=w219, "Message"="Are you sure you want to change the AFM Type? Doing so may cause problems.") -> ("error out"=w218:errorcluster, "OK?"=w220:bool)  [unwired: 8 in]
                n85 = Select(t=w223, s=w220, f=w222) -> (s? t:f=w221:u16)
                n86 = local write "AFM Type"(w221) -> ()
                n87 = Select(t="Litho: Refresh Render\nUI: IMAQ Render" ("State(s) at Back (\"\")"), s=w220, f="" ("Empty String Constant")) -> (s? t:f=w224:string)
                n88 = call <vilib>:"Add State(s) to Queue__jki_lib_state_machine.vi"("State(s) in (\"\")"=w227, "State(s) at Back (\"\")"=w224) -> ("States Out"=w228:string)  [unwired: 13 in]
              }
              event "Done": Value Change {
                n89 = event-data() -> ()  [unwired: 1 in, 6 out]
                n90 = Select(t="Macro: Exit", s="Done", f="" ("Empty String Constant")) -> (s? t:f=w230:string)
                n91 = call <vilib>:"Add State(s) to Queue__jki_lib_state_machine.vi"("State(s) in (\"\")"=w234, "State(s) at Back (\"\")"=w230) -> ("States Out"=w235:string)  [unwired: 13 in]
              }
              event "Image Data Range": Value Change {
                # "Note: This event is modified to only allow a single event in the event queue, which should be the most recent one. This keeps the UI snappy when switching the Image Data Range."
                n92 = event-data() -> ()  [unwired: 1 in, 6 out]
                n93 = call <vilib>:"Add State(s) to Queue__jki_lib_state_machine.vi"("State(s) in Front (\"\")"="Litho: Load Background\nLitho: Display Background\nLitho: Refresh Render\nUI: IMAQ Render", "State(s) in (\"\")"=w239) -> ("States Out"=w240:string)  [unwired: 13 in]
              }
              event "Save Render": Value Change {
                n94 = event-data() -> ()  [unwired: 1 in, 6 out]
                n95 = Unbundle By Name(w254) -> ("IMAQ (Work)"=w252:T1)
                n96 = call "File Dialog"("prompt"="Select a filename to save render as", "error in"=w246, "pattern (all files)"="*.png", "pattern label"="Portable Network Graphics") -> ("selected path"=w249:path, "error out"=w244:errorcluster)  [unwired: 8 in, 2 out]
                n97 = call "IMAQ Merge Overlay"("error in (no error)"=w244, "Image Src"=w252) -> ("error out"=w253:errorcluster, "Image Dst Out"=w251:T1)  [unwired: 8 in]
                n98 = call-poly "IMAQ Write File 2"("error in (no error)"=w253, "File Path"=w249, "Image"=w251) -> ("error out"=w250:errorcluster)  [unwired: 7 in, 1 out]
                n99 = call <vilib>:"Add State(s) to Queue__jki_lib_state_machine.vi"("State(s) in Front (\"\")"="UI: Status >> Save Render" ("State(s) in Front (\"\")"), "State(s) in (\"\")"=w255) -> ("States Out"=w256:string)  [unwired: 13 in]
              }
              event "Run": Value Change {
                n100 = event-data() -> ()  [unwired: 1 in, 6 out]
                n101 = call <vilib>:"Add State(s) to Queue__jki_lib_state_machine.vi"("State(s) in Front (\"\")"="UI: Status >> RUN\nUI: Enable Run >> Disabled\nDriver: Run Lithography", "State(s) in (\"\")"=w258) -> ("States Out"=w259:string)  [unwired: 13 in]
              }
              event "Abort": Value Change {
                # "We will make abort notifier = True"
                n102 = event-data() -> ()  [unwired: 1 in, 6 out]
                n103 = Unbundle By Name(w265) -> ("AFM_Driver_Manager"=w269:refnum<class "AFM_Driver_Manager.lvclass">)
                n104 = call "AFM_Driver_Manager.Abort.vi"("AFM_Driver_Manager in"=w269) -> ("error out"=w263:errorcluster, "AFM_Driver_Manager out"=w264:refnum<class "AFM_Driver_Manager.lvclass">)  [unwired: 9 in]
                n105 = disable-structure "Diagram Disable Structure" shown="Disabled" {
                  disable-tunnel: w263 -> [w272 _]
                  frame Disabled {
                    n106 = call "Display Message to User3"("error in (no error)"=w272) -> ()  [unwired: 9 in, 2 out]
                  }
                  frame Enabled {
                  }
                }
                n107 = Bundle By Name(cluster=w265, "AFM_Driver_Manager"=w264) -> (w266:T20)
                n108 = Merge Errors(w267, w263) -> (w268:errorcluster)
                n109 = call <vilib>:"Add State(s) to Queue__jki_lib_state_machine.vi"("State(s) in Front (\"\")"="UI: Enable Run >> Enabled\nUI: Status >> ABORT", "State(s) in (\"\")"=w270) -> ("States Out"=w271:string)  [unwired: 13 in]
              }
              event User Event {
                # "Destroy the abort notifier"
                # "Set Run Button to False when finished with lithography"
                n110 = event-data() -> ()  [unwired: 1 in, 5 out]
                n111 = disable-structure "Diagram Disable Structure" shown="Disabled" {
                  frame Disabled {
                    n112 = call "Display Message to User2"() -> ()  [unwired: 10 in, 2 out]
                  }
                  frame Enabled {
                  }
                }
                n113 = Unbundle By Name(w277) -> ("AFM_Driver_Manager"=w281:refnum<class "AFM_Driver_Manager.lvclass">)
                n114 = call "AFM_Driver_Manager.OnLithographyFinish.vi"("error in (no error)"=w278, "AFM_Driver_Manager in"=w281) -> ("error out"=w275:errorcluster, "AFM_Driver_Manager out"=w279:refnum<class "AFM_Driver_Manager.lvclass">)  [unwired: 8 in]
                n115 = control-ref of="Run"() -> (w283:refnum<vi>)
                n116 = Bundle By Name(cluster=w277, "AFM_Driver_Manager"=w279) -> (w280:T20)
                n117 = property on="Property Node" class="Bool (strict)"(reference=w283, "Value"=FALSE) -> (error out=w276:errorcluster)  [unwired: 1 in, 1 out]
                n118 = Merge Errors(w275, w276) -> (w274:errorcluster)
                n119 = call <vilib>:"Add State(s) to Queue__jki_lib_state_machine.vi"("State(s) in Front (\"\")"="UI: Enable Run >> Enabled\nUI: Status >> Lithography Process Finished" ("State(s) in Front (\"\")"), "State(s) in (\"\")"=w284) -> ("States Out"=w285:string)  [unwired: 13 in]
              }
              event "Help": Value Change {
                n120 = event-data() -> ()  [unwired: 1 in, 6 out]
                n121 = call-poly <vilib>:"Open URL in Default Browser.vi"("error in (no error)"=w292, "URL"="https://github.com/levylabpitt/AFM-Lithography") -> ("error out"=w291:errorcluster)  [unwired: 4 in, 1 out]
                n122 = call <vilib>:"Add State(s) to Queue__jki_lib_state_machine.vi"("State(s) in Front (\"\")"="UI: Status >> HELP" ("State(s) in Front (\"\")"), "State(s) in (\"\")"=w287) -> ("States Out"=w288:string)  [unwired: 13 in]
              }
              event "Inkscape File (.svg)": Value Change {
                n123 = event-data() -> ("NewVal"=w298:path)  [unwired: 1 in, 5 out]
                n124 = Bundle By Name(cluster=w299, "Inkscape File (.svg)"=w298) -> (w300:T20)
                n125 = call <vilib>:"Build State String with Arguments__JKI_lib_State_Machine.vi"("Arguments (\"\")"="Inkscape File Changed" ("Arguments (\"\")"), "State"="UI: Status") -> ("State with Arguments"=w297:string)  [unwired: 4 in]
                n126 = call <vilib>:"Add State(s) to Queue__jki_lib_state_machine.vi"("State(s) in Front (\"\")"=w297, "State(s) in (\"\")"="UI: Ready >> FALSE\nMacro: Refresh\n//Macro: Send Driver\nConfiguration: Write\nUI: Ready >> TRUE") -> ("States Out"=w293:string)  [unwired: 13 in]
                n127 = call <vilib>:"Add State(s) to Queue__jki_lib_state_machine.vi"("State(s) in Front (\"\")"=w293, "State(s) in (\"\")"=w302) -> ("States Out"=w301:string)  [unwired: 13 in]
              }
              event "Autosave?": Value Change {
                n128 = event-data() -> ("NewVal"=w309:bool)  [unwired: 1 in, 5 out]
                n129 = Bundle By Name(cluster=w310, "Autosave?"=w309) -> (w311:T20)
                n130 = Select(t="UI: Autosave Render", s=w309, f="") -> (s? t:f=w308:string)
                n131 = call <vilib>:"Add State(s) to Queue__jki_lib_state_machine.vi"("State(s) in Front (\"\")"="Configuration: Write" ("State(s) in Front (\"\")"), "State(s) in (\"\")"=w308) -> ("States Out"=w304:string)  [unwired: 13 in]
                n132 = call <vilib>:"Add State(s) to Queue__jki_lib_state_machine.vi"("State(s) in Front (\"\")"=w304, "State(s) in (\"\")"=w313) -> ("States Out"=w312:string)  [unwired: 13 in]
              }
              event "Autosave Path": Value Change {
                n133 = event-data() -> ("NewVal"=w322:path)  [unwired: 1 in, 5 out]
                n134 = Bundle By Name(cluster=w323, "Autosave Path"=w322) -> (w316:T20)
                n135 = Unbundle By Name(w316) -> ("Autosave?"=w315:bool)
                n136 = Select(t="UI: Autosave Render", s=w315, f="") -> (s? t:f=w321:string)
                n137 = call <vilib>:"Add State(s) to Queue__jki_lib_state_machine.vi"("State(s) in Front (\"\")"="Configuration: Write" ("State(s) in Front (\"\")"), "State(s) in (\"\")"=w321) -> ("States Out"=w317:string)  [unwired: 13 in]
                n138 = call <vilib>:"Add State(s) to Queue__jki_lib_state_machine.vi"("State(s) in Front (\"\")"=w317, "State(s) in (\"\")"=w325) -> ("States Out"=w324:string)  [unwired: 13 in]
              }
              event "Background Image": Value Change {
                n139 = event-data() -> ("NewVal"=w327:path)  [unwired: 1 in, 5 out]
                n140 = Bundle By Name(cluster=w328, "Background Image"=w327) -> (w329:T20)
                n141 = call <vilib>:"Add State(s) to Queue__jki_lib_state_machine.vi"("State(s) in Front (\"\")"="UI: Status >> Background Image Changed\nUI: Ready >> FALSE\nLitho: Load Background\nLitho: Display Background\nLitho: Refresh Render\nUI: IMAQ Render\nDriver: Background Image\nUI: Ready >> TRUE\nConfiguration: Write", "State(s) in (\"\")"=w332) -> ("States Out"=w331:string)  [unwired: 13 in]
              }
              event "Create Overlay": Value Change {
                n142 = event-data() -> ()  [unwired: 1 in, 6 out]
                n143 = call <vilib>:"Add State(s) to Queue__jki_lib_state_machine.vi"("State(s) in Front (\"\")"="UI: Status >> Create Overlay\nUI: Ready >> FALSE\nUI: Overlay\nUI: Ready >> TRUE", "State(s) in (\"\")"=w337) -> ("States Out"=w336:string)  [unwired: 13 in]
              }
              event "Page": Value Change {
                n144 = event-data() -> ()  [unwired: 1 in, 6 out]
                n145 = call <vilib>:"Add State(s) to Queue__jki_lib_state_machine.vi"("State(s) in Front (\"\")"="UI: Status >> Image Page Changed\nUI: Ready >> FALSE\nLitho: Load Background\nLitho: Display Background\nLitho: Refresh Render\nUI: IMAQ Render\nUI: Ready >> TRUE", "State(s) in (\"\")"=w342) -> ("States Out"=w341:string)  [unwired: 13 in]
              }
              event "Refresh Button": Value Change {
                n146 = event-data() -> ()  [unwired: 1 in, 6 out]
                n147 = call <vilib>:"Add State(s) to Queue__jki_lib_state_machine.vi"("State(s) in Front (\"\")"="UI: Status >> REFRESH\nUI: Ready >> FALSE\nMacro: Refresh\nMacro: Send Driver\nUI: Ready >> TRUE", "State(s) in (\"\")"=w347) -> ("States Out"=w346:string)  [unwired: 13 in]
              }
              event "Patterns": Value Change {
                n148 = event-data() -> ()  [unwired: 1 in, 6 out]
                n149 = call <vilib>:"Add State(s) to Queue__jki_lib_state_machine.vi"("State(s) in (\"\")"=w351, "State(s) at Back (\"\")"="UI: Status >> New Active Object Selected\nUI: Update Subpanel\nLitho: Order Data\nDriver: Litho Data" ("State(s) at Back (\"\")")) -> ("States Out"=w350:string)  [unwired: 13 in]
              }
              event "MCLB": Value Change {
                n150 = event-data() -> ("NewVal"=w356:i32)  [unwired: 1 in, 5 out]
                n151 = Unbundle By Name(w358) -> ("MCLB"=w360:refnum<class "Selector.lvclass">)
                n152 = call-dynamic "Write Value.vi"("error in (no error)"=w354, "Value"=w356, "Selector in"=w360) -> ("error out"=w355:errorcluster, "Selector out"=w357:refnum<class "Selector.lvclass">)  [unwired: 7 in]
                n153 = Bundle By Name(cluster=w358, "MCLB"=w357) -> (w359:T20)
                n154 = call <vilib>:"Add State(s) to Queue__jki_lib_state_machine.vi"("State(s) in (\"\")"=w362) -> ("States Out"=w361:string)  [unwired: 14 in]
              }
              event "MCLB": Shortcut Menu Activation? {
                n155 = event-data() -> ("MenuRef"=w371:refnum<k9>, "Coords"=w370:T22)  [unwired: 1 in, 5 out]
                n156 = Unbundle By Name(w368) -> ("MCLB"=w367:refnum<class "Selector.lvclass">)
                n157 = disable-structure shown="Enabled" {
                  disable-tunnel: w371 -> [w379 _]
                  disable-tunnel: w370 -> [w378 _]
                  disable-tunnel: w367 -> [w377 w381]
                  disable-tunnel: [w376 w381] -> w366
                  disable-tunnel: [w375 w380] -> w365
                  disable-tunnel: w364 -> [w374 w380]
                  frame Disabled {
                    n158 = call-dynamic "Populate Menu Activation.vi"("error in (no error)"=w374, "Point32"=w378, "MenuRef"=w379, "Selector in"=w377) -> ("error out"=w375:errorcluster, "Selector out"=w376:refnum<class "Selector.lvclass">)  [unwired: 6 in]
                  }
                  frame Enabled {
                  }
                }
                n159 = Bundle By Name(cluster=w368, "MCLB"=w366) -> (w369:T20)
                n160 = event-data("Discard?"=FALSE) -> ()  [unwired: 1 in, 1 out]
                n161 = call <vilib>:"Add State(s) to Queue__jki_lib_state_machine.vi"("State(s) in (\"\")"=w373) -> ("States Out"=w372:string)  [unwired: 14 in]
              }
              event "MCLB": Shortcut Menu Selection (User) {
                n162 = event-data() -> ("ItemPath"=w383:string)  [unwired: 1 in, 7 out]
                n163 = Bundle By Name(cluster=w387, "Menu Path"=w383) -> (w388:T20)
                n164 = Match Pattern(string=w383, regular expression="\\:") -> (before substring=w384:string)  [unwired: 1 in, 3 out]
                n165 = call <vilib>:"Build State String with Arguments__JKI_lib_State_Machine.vi"("Arguments (\"\")"=w384, "State"="MCLB: SCM Selection") -> ("State with Arguments"=w382:string)  [unwired: 4 in]
                n166 = call <vilib>:"Add State(s) to Queue__jki_lib_state_machine.vi"("State(s) in Front (\"\")"=w382, "State(s) in (\"\")"=w390) -> ("States Out"=w389:string)  [unwired: 13 in]
              }
              event "MCLB": Mouse Down? {
                n167 = event-data() -> ("Coords"=w400:T22, "Button"=w399:u16, "PlatMods"=w395:T23)  [unwired: 1 in, 5 out]
                n168 = Unbundle By Name(w403) -> ("MCLB"=w405:refnum<class "Selector.lvclass">)
                n169 = disable-structure shown="Enabled" {
                  disable-tunnel: w405 -> [w418 w432]
                  disable-tunnel: [w417 w432] -> w404
                  disable-tunnel: w400 -> [w416 _]
                  disable-tunnel: w399 -> [w415 _]
                  disable-tunnel: [w414 w431] -> w398
                  disable-tunnel: w397 -> [w413 w431]
                  disable-tunnel: [w412 _] -> w396
                  disable-tunnel: w395 -> [w411 _]
                  disable-tunnel: [w410 _] -> w394
                  disable-tunnel: ["Database: Update Enable" _] -> w393
                  frame Disabled {
                    n170 = Bundle By Name(cluster=T4 {"Point"={"Left"=0, "Top"=0}, "Button"=0, "PlatMods"={"Shift"=FALSE, "Ctrl"=FALSE, "Alt"=FALSE, "Cmd"=FALSE, "Opt"=FALSE}} ("Event Data"), "Point"=w416, "Button"=w415, "PlatMods"=w411) -> (w419:T4)
                    n171 = call-dynamic "Handle Mouse Down.vi"("error in (no error)"=w413, "Event Data"=w419, "Selector in"=w418) -> ("error out"=w421:errorcluster, "Enable Change"=w412:bool, "Selector out"=w420:refnum<class "Selector.lvclass">)  [unwired: 6 in]
                    n172 = case shown="True" w412 {
                      tunnel: w420 -> [w425 w430]
                      tunnel: w421 -> [w424 w429]
                      tunnel: [w424 w428] -> w414
                      tunnel: [w425 w427] -> w417
                      tunnel: ["" ("Name") w426] -> w410
                      frame False {
                      }
                      frame True {
                        n173 = call "Change Active Enable Symbol.vi"("error in (no error)"=w429, "Selector in"=w430) -> ("error out"=w428:errorcluster, "Name"=w426:string, "Selector out"=w427:refnum<class "Selector.lvclass">)  [unwired: 7 in]
                      }
                    }
                  }
                  frame Enabled {
                  }
                }
                n174 = Bundle By Name(cluster=w403, "MCLB"=w404) -> (w402:T20)
                n175 = call <vilib>:"Build State String with Arguments__JKI_lib_State_Machine.vi"("Arguments (\"\")"=w394, "State"=w393) -> ("State with Arguments"=w392:string)  [unwired: 4 in]
                n176 = Select(t=w392, s=w396, f="") -> (s? t:f=w401:string)
                n177 = event-data("Discard?"=w396) -> ()  [unwired: 4 in, 1 out]
                n178 = call <vilib>:"Add State(s) to Queue__jki_lib_state_machine.vi"("State(s) in Front (\"\")"=w401, "State(s) in (\"\")"=w408) -> ("States Out"=w407:string)  [unwired: 13 in]
              }
              event "MCLB": Drag Ended {
                n179 = event-data() -> ("CtlRef"=w437:refnum<vi>)  [unwired: 1 in, 4 out]
                n180 = property class="MCListbox (strict)"(reference=w437) -> ("ItemNames"=w434:string[][])  [unwired: 1 in, 2 out]
                n181 = Bundle By Name(cluster=w435, "Item Names"=w434) -> (w436:T20)
                n182 = call <vilib>:"Add State(s) to Queue__jki_lib_state_machine.vi"("State(s) in Front (\"\")"="MCLB: Reorder", "State(s) in (\"\")"=w439) -> ("States Out"=w438:string)  [unwired: 13 in]
              }
              event "MCLB": Drag Starting {
                n183 = event-data() -> ()  [unwired: 1 in, 10 out]
                n184 = call <vilib>:"Add State(s) to Queue__jki_lib_state_machine.vi"("State(s) in (\"\")"=w443, "State(s) at Back (\"\")"="UI: Status >> New Active Object Selected\nUI: Update Subpanel\nLitho: Order Data\nDriver: Litho Data" ("State(s) at Back (\"\")")) -> ("States Out"=w442:string)  [unwired: 13 in]
              }
              event "Patterns": Drag Starting {
                n185 = event-data() -> ("CtlRef"=w451:refnum<vi>)  [unwired: 1 in, 9 out]
                n186 = property class="LstBox (strict)"(reference=w451, error in=w447) -> (error out=w446:errorcluster, "Item Names"=w448:string[])  [unwired: 1 out]
                n187 = Bundle By Name(cluster=w449, "Drag and Drop.Start"=w448) -> (w450:T20)
                n188 = call <vilib>:"Add State(s) to Queue__jki_lib_state_machine.vi"("State(s) in (\"\")"=w453) -> ("States Out"=w452:string)  [unwired: 14 in]
              }
              event "Patterns": Drag Ended {
                n189 = event-data() -> ("CtlRef"=w462:refnum<vi>)  [unwired: 1 in, 4 out]
                n190 = property class="LstBox (strict)"(reference=w462) -> ("Item Names"=w455:string[])  [unwired: 1 in, 2 out]
                n191 = Unbundle By Name(w460) -> ("Drag and Drop.Start"=w459:string[])
                n192 = Equal?(x=w459, y=w455) -> (x = y?=w458:bool)
                n193 = Select(t="" ("State(s) in Front (\"\")"), s=w458, f="//Listbox: Compare Values\nListbox: Reorder Data\n//Litho: Order Data\nDriver: Litho Data\nLitho: Refresh Render") -> (s? t:f=w454:string)
                n194 = Bundle By Name(cluster=w460, "Drag and Drop.Working"=w455, "Drag and Drop.Running"=w455) -> (w461:T20)
                n195 = call <vilib>:"Add State(s) to Queue__jki_lib_state_machine.vi"("State(s) in Front (\"\")"=w454, "State(s) in (\"\")"=w464) -> ("States Out"=w463:string)  [unwired: 13 in]
              }
              event Panel Close? {
                # "Discard the event because we'll close the front panel ourselves in Macro: Exit"
                # "Close Panel button (pressed) Event\n(this executes Macro: Exit to terminate the VI)"
                n196 = event-data() -> ()  [unwired: 1 in, 1 out]
                n197 = event-data ("Event Filter Node")("Discard?"=TRUE) -> ()  [unwired: 1 in, 1 out]
                n198 = call <vilib>:"Add State(s) to Queue__jki_lib_state_machine.vi"("State(s) in Front (\"\")"="Macro: Exit", "State(s) in (\"\")"=w470) -> ("States Out"=w469:string)  [unwired: 13 in]
              }
            }
          }
          frame "---------- Core ----------" {
            # "Do not put any code in this frame.\n(it is a separator no-op)"
            n199 = call <vilib>:"Add State(s) to Queue__jki_lib_state_machine.vi"("State(s) in (\"\")"=w474) -> ("States Out"=w475:string)  [unwired: 14 in]
          }
          frame Default {
            w484 = 42 items=["No error", "Argument error", "Memory is full", "Out of zone", "End of file", "File already open", "Generic file I/O error", "File not found", "File permission error", "Disk is full", "Duplicate path", "Too many files open", "System feature not enabled", "Resource file not found", "Cannot add resource", "Resource not found", "Image not found", "Image memory error", "Pen does not exist", "Config type invalid", "Config token not found", "Config parse error", "Config memory error", "Bad external code format", "Bad external code offset", "External code not present", "Null window", "Destroy window error", "Null menu", "Print aborted", "Bad print record", "Print driver error", "Windows error during printing", "Memory error during printing", "Print dialog error", "Generic print error", "Invalid device refnum", "Device not found", "Device parameter error", "Device unit error", "Cannot open device", "Device call aborted", "Generic error", "Cancelled by user", "Object ID too low", "Object ID too high", "Object not in heap", "Unknown heap", "Unknown object (invalid DefProc)", "Unknown object (DefProc not in table)", "Message out of range", "Invalid (null) method", "Unknown message", "Manager call not supported", "Bad address", "Network operation in progress", "Network operation timed out", "Connection is busy", "Network attribute not supported", "Network error", "Address in use", "System out of memory", "Connection aborted", "Connection refused", "Not connected", "Already connected", "Connection closed", "Initialization error (interapplication manager)", "Bad occurrence", "Wait on unbound occurrence handler", "Occurrence queue overflow", "Datalog type conflict", "Unused", "Unrecognized type (interapplication manager)", "Memory corrupt", "Failed to make temporary DLL", "Old CIN version", "Drag socket not found", "Failed to load drop-object", "Failed to register OLE object", "Failed to release OLE object", "Format specifier type mismatch", "Unknown format specifier", "Too few format specifiers", "Too many format specifiers", "Scan failed", "Newer CIN version", "Error converting to variant", "Runtime menu error", "Password tampered", "Variant attribute not found", "Incompatible variant data type", "Event data is not available", "Event Store is not present", "Occurrence is not found", "Event Queue is not created", "Event info is not available", "Refnum passed is NULL", "Error retrieving Class GUID", "Error retrieving CoClass GUID", "Error retrieving TypeLib GUID.", "Bad built application magic bytes.", "Specific driver is different from the specific driver associated with the Logical Name.", "There is no session opened to the class driver.", "Max Error", "MAX - Error with config objects", "MAX - Error loading configuration", "MAX - Group not supported"]
            # "State Syntax:\nStateCategory: State >> Argument\nLine Terminator: Line feed\nExample:\nUI: Help >> About\n\nWhere \"UI\" is the state category\nWhere \"Help\" is the state\nWhere \"About\" is the argument\nOther Examples:\nApp Data: Initialize\nUI: Initialize\nHelp >> About\n\nCommenting:\nTo add a comment use \"//\" or \"#\" and all text to the right will be ignored\nCommenting Example:\nUI: Initialize // This initializes the UI\n# This whole line is a comment\n// Another comment line"
            # "For instructions on how to use the JKI State Machine, examples and video tutorials, visit:\nhttp://jki.net/state-machine/\n\nJKI State Machine™\nhttp://jki.net/state-machine/\nCopyright (C) 2005-2018, JKI <info@jki.net>\nALL RIGHTS RESERVED"
            # "Handle mistyped state name (developer tool)"
            # "Current State"
            # "Do not delete, rename, or modify this frame.\n(this is used to capture unhandled states and typos)"
            n200 = Format Into String(format string="Software Exception: Unhandled State \"%s\"." ("message"), error in=w486, w478) -> (resulting string=w483:string, error out=w488:errorcluster)  [unwired: 1 in]
            n201 = call <vilib>:"Error Cluster From Error Code.vi"("show call chain? (False)"=TRUE, "error in (no error)"=w488, "error message (\"\")"=w483, "error code (0)"=w484) -> ("error out"=w487:errorcluster)  [unwired: 5 in]
            n202 = call <vilib>:"Add State(s) to Queue__jki_lib_state_machine.vi"("State(s) in (\"\")"=w481) -> ("States Out"=w482:string)  [unwired: 14 in]
          }
          frame "Initialize Core Data" {
            # "Do not delete, rename, or modify this frame.\n(this is used to determine panel behavior on exit)"
            # "originally closed?"
            # "exe?"
            # "If panel starts closed or is an EXE, then close it when we exit"
            n203 = property on="Property Node" class="VI"() -> ("Front Panel.Open"=w499:bool)  [unwired: 2 in, 2 out]
            n204 = property on="Property Node" class="App"() -> ("App.Kind"=w498:T5)  [unwired: 2 in, 2 out]
            n205 = control-ref of="Current VI Reference"() -> (w496:refnum<vi>)
            n206 = Not(x=w499) -> (.not. x?=w492:bool)
            n207 = Equal?(x=w498, y=T5."Run Time System" ("Application:Kind")) -> (x = y?=w491:bool)
            n208 = Or(x=w492, y=w491) -> (x .or. y?=w497:bool)
            n209 = Bundle By Name(cluster=w494, "Core.Current VI Reference"=w496, "Core.Close Panel on Exit?"=w497) -> (w493:T20)
            n210 = call <vilib>:"Add State(s) to Queue__jki_lib_state_machine.vi"("State(s) in (\"\")"=w495) -> ("States Out"=w500:string)  [unwired: 14 in]
          }
          frame "Error Handler" {
            # "Unhandled Error -- Display it"
            # "Handle any errors here.\nYou can also output any states to clean-up after errors occur"
            # "Clear error"
            n211 = call <vilib>:"General Error Handler.vi"("[error source] (\" \")"=w505, "error in (no error)"=w509) -> ()  [unwired: 9 in, 5 out]
            n212 = call <vilib>:"Add State(s) to Queue__jki_lib_state_machine.vi"("State(s) in Front (\"\")"="/* Post Error States", "State(s) in (\"\")"=w504) -> ("States Out"=w507:string)  [unwired: 13 in]
          }
          frame "Exit" {
            # "Do not put any code in this frame.\n(No errors that occur here will be handled.)"
            n213 = call <vilib>:"Add State(s) to Queue__jki_lib_state_machine.vi"("State(s) in (\"\")"=w511) -> ("States Out"=w514:string)  [unwired: 14 in]
          }
          frame "---------- Data ----------" {
            # "Do not put any code in this frame.\n(It is a separator no-op. You can make a copy of this frame to create a new Data frame)"
            n214 = call <vilib>:"Add State(s) to Queue__jki_lib_state_machine.vi"("State(s) in (\"\")"=w518) -> ("States Out"=w519:string)  [unwired: 14 in]
          }
          frame "Data: Initialize" {
            w521 = string[][] []  # Item Names
            w522 = ""  # Menu Path
            w528 = refnum<class "Tool Data.lvclass"> refnum  # Tooler
            w529 = T24 {"paths"=[], "funnels"=[], "rects"=[], "dots"=[]}  # IDs
            w542 = T25 {"Start"=[], "End"=[], "Running"=[], "Working"=[]}  # Drag and Drop
            w543 = refnum<class "Configuration.lvclass"> refnum  # Config
            w527 = ""  # Status
            w530 = cluster{dbl, dbl} {100.0, 0.0}  # Image Data Range
            w531 = FALSE  # Hide Labels
            w532 = refnum<class "Setting Database.lvclass"> refnum  # Database
            w535 = refnum<class "ParseVectorFile.lvclass"> refnum  # ParseVectorFile
            w536 = T1 refnum  # IMAQ (Work)
            w537 = refnum<class "AFM_Driver_Manager.lvclass"> refnum  # AFM_Driver_Manager
            w538 = path ""  # root path
            w541 = T26 {"paths"=[], "funnels"=[], "rects"=[], "Dots"=[]}  # Parsing Data
            w539 = refnum<vi>[] []  # VI Refs
            w540 = T27 []  # Lithography Data
            w550 = T28 {"Current VI Reference"=refnum, "Close Panel on Exit?"=FALSE}  # Core
            # "Initialize the shift-register data, here.\n(data names are defined by what you wire into the bundle function)"
            n215 = control-ref of="MCLB"() -> (w525:refnum<vi>)
            n216 = call "Constructor.vi"("error in (no error)"=w523, "Reference"=w525) -> ("error out"=w524:errorcluster, "MCLB"=w526:refnum<class "Selector.lvclass">)  [unwired: 8 in]
            n217 = Bundle("Core"=w550, "Parsing Data"=w541, "Lithography Data"=w540, "VI Refs"=w539, "root path"=w538, "AFM_Driver_Manager"=w537, "IMAQ (Work)"=w536, "Background Image"=w545, "Inkscape File (.svg)"=w544, "ParseVectorFile"=w535, "Database"=w532, "Hide Labels"=w531, "Autosave?"=w534, "Autosave Path"=w533, "Image Data Range"=w530, "Status"=w527, "Config"=w543, "Drag and Drop"=w542, "IDs"=w529, "Tooler"=w528, "MCLB"=w526, "Menu Path"=w522, "Item Names"=w521) -> (w547:T20)  [unwired: 1 in]
            n218 = call <vilib>:"Add State(s) to Queue__jki_lib_state_machine.vi"("State(s) in (\"\")"=w548) -> ("States Out"=w549:string)  [unwired: 14 in]
          }
          frame "Data: Run Edit VIs" {
            w552 = path[] [path "subVIs/subpanel/Path Edit.vi", path "subVIs/subpanel/Rect Edit.vi", path "subVIs/subpanel/Funnel Edit.vi", path "subVIs/subpanel/Dot Edit.vi"]  # Edit VIs
            # "#via_ignore Unused Code"
            # "Is this supposed to be unwired?"
            n219 = Unbundle By Name(w554) -> ("root path"=w553:path)
            n220 = for {
              tunnel: w553 -> [w562]
              tunnel: w552 -> [w561] mode=indexing
              tunnel: [w560] -> _ mode=indexing
              n221 = Build Path(base path=w562, name or relative path=w561) -> (appended path=w560:path)
            }
            n222 = for {
              tunnel: [w564] -> w556 mode=indexing
              shift-right: [w567] -> w558
              shift-left: w559 -> [w568]
              tunnel: w552 -> [w563] mode=indexing
              # "Load and run Plugin VIs"
              n223 = Open VI Reference(vi path=w563, error in (no error)=w568) -> (vi reference=w565:refnum<vi>, error out=w569:errorcluster)  [unwired: 4 in]
              n224 = invoke on="Invoke Node" class="VI" method="Run VI"(reference=w565, error in=w569, "Wait until done"=FALSE ("Wait Until Done")) -> (reference out=w564:refnum<vi>, error out=w567:errorcluster)  [unwired: 2 in, 3 out]
            }
            n225 = Bundle By Name(cluster=w554, "VI Refs"=w556) -> (w557:T20)
          }
          frame "Data: Set Root Path" {
            # "For built exes, this will provide the path inside the exe for this VI, and we can use this as a relative path. For unbuilt environments, it provides the path of the VI running it. Since we dont care about this path of this VI, we strip it.\n\nIn other words, this provides a more consistent way to generate relative paths for both exes and development environments."
            # "Do not put any code in this frame.\n(It is a separator no-op. You can make a copy of this frame to create a new Data frame)"
            n226 = call <userlib>:"Current VI's Path__ogtk.vi"() -> ("Current VI's Path (+ Relative)"=w572:path)  [unwired: 1 in]
            n227 = Strip Path(path=w572) -> (stripped path=w571:path)  [unwired: 1 out]
            n228 = Bundle By Name(cluster=w573, "root path"=w571) -> (w574:T20)
            n229 = call <vilib>:"Add State(s) to Queue__jki_lib_state_machine.vi"("State(s) in (\"\")"=w575) -> ("States Out"=w576:string)  [unwired: 14 in]
          }
          frame "Data: Cleanup" {
            # "Cleanup any data and references, here.\n(this is called automatically, by the Macro: Exit)"
            n230 = Unbundle By Name(w586) -> ("Core.Current VI Reference"=w587:refnum<vi>, "VI Refs"=w588:refnum<vi>[], "IMAQ (Work)"=w581:T1)
            n231 = call "IMAQ Dispose"("All Images? (No)"=TRUE, "Image"=w581, "error in (no error)"=w579) -> ("error out"=w578:errorcluster)  [unwired: 3 in]
            n232 = invoke on="AFM Settings" class="SubPnl" method="Remove VI"(error in=w578) -> (error out=w583:errorcluster)  [unwired: 2 in, 2 out]
            n233 = for {
              tunnel: w588 -> [w591] mode=indexing
              shift-right: [w592] -> w584
              shift-left: w583 -> [w593]
              n234 = call "Abort If Not Refnum.vi"("error in (no error)"=w593, "VI in"=w591) -> ("error out"=w592:errorcluster)  [unwired: 9 in]
            }
            n235 = Close Reference(reference=w587, error in (no error)=w584) -> (error out=w590:errorcluster)
            n236 = call <vilib>:"Add State(s) to Queue__jki_lib_state_machine.vi"("State(s) in (\"\")"=w585) -> ("States Out"=w589:string)  [unwired: 14 in]
          }
          frame "---------- Events ----------" {
            # "Do not put any code in this frame.\n(It is a separator no-op. You can make a copy of this frame to create a new UI frame)"
            n237 = call <vilib>:"Add State(s) to Queue__jki_lib_state_machine.vi"("State(s) in (\"\")"=w596) -> ("States Out"=w597:string)  [unwired: 14 in]
          }
          frame "Events: Register" {
            # "Do not put any code in this frame.\n(It is a separator no-op. You can make a copy of this frame to create a new UI frame)"
            n238 = Unbundle By Name(w602) -> ("AFM_Driver_Manager"=w608:refnum<class "AFM_Driver_Manager.lvclass">, "Database"=w601:refnum<class "Setting Database.lvclass">)
            n239 = call "Setting Database.GetPublicEvents.vi"("Setting Database"=w601) -> ("error out"=w599:errorcluster, "Public Events"=w600:T29)  [unwired: 8 in, 1 out]
            n240 = call "AFM_Driver_Manager.GetPublicEvents.vi"("AFM_Driver_Manager in"=w608) -> ("error out"=w603:errorcluster, "AFM_Driver Events"=w607:T30)  [unwired: 8 in, 1 out]
            n241 = register-events(w607, w600) -> (reference out=w609:refnum<event-registration>, error out=w606:errorcluster)  [unwired: 2 in]
            n242 = Merge Errors(w604, w606, w603, w599) -> (w605:errorcluster)
            n243 = call <vilib>:"Add State(s) to Queue__jki_lib_state_machine.vi"("State(s) in (\"\")"=w610) -> ("States Out"=w611:string)  [unwired: 14 in]
          }
          frame "Events: Unregister" {
            # "Do not put any code in this frame.\n(It is a separator no-op. You can make a copy of this frame to create a new UI frame)"
            n244 = Unregister For Events(event registration refnum=w614, error in=w613) -> (error out=w612:errorcluster)
            n245 = call <vilib>:"Add State(s) to Queue__jki_lib_state_machine.vi"("State(s) in (\"\")"=w616) -> ("States Out"=w617:string)  [unwired: 14 in]
          }
          frame "---------- UI ----------" {
            # "Do not put any code in this frame.\n(It is a separator no-op. You can make a copy of this frame to create a new UI frame)"
            n246 = call <vilib>:"Add State(s) to Queue__jki_lib_state_machine.vi"("State(s) in (\"\")"=w620) -> ("States Out"=w621:string)  [unwired: 14 in]
          }
          frame "UI: Initialize" {
            # "Initialize the User Interface, here.\n(this is called automatically, by the Macro: Init)"
            n247 = call <userlib>:"MGI Get Executable Version.vi"() -> ("Version"=w626:string)  [unwired: 7 in]
            n248 = Format Into String(format string="v%s", w626) -> (resulting string=→"version":string)  [unwired: 2 in, 1 out]
            n249 = control-ref of="Image Data Range"() -> (w633:refnum<vi>)
            n250 = disable-structure shown="TARGET_TYPE==RT" {
              frame condition #0 {
                n251 = local write "Settings"(T6."Program Settings" ("Settings")) -> ()
              }
              frame condition #1 (active) {
              }
            }
            n252 = property class="Slide (strict)"(reference=w633, error in=w628, "ShowValTip"=FALSE) -> (error out=w630:errorcluster)  [unwired: 1 out]
            n253 = property on="Hide Labels?" class="Bool (strict)"("Value"=FALSE ("Hide Labels?")) -> ()  [unwired: 2 in, 2 out]
            n254 = call <userlib>:"Fit VI window to Largest Dec__ogtk.vi"("error in (no error)"=w628) -> ("error out"=w629:errorcluster)  [unwired: 5 in, 1 out]
            n255 = Merge Errors(w630, w629) -> (w631:errorcluster)
            n256 = call <vilib>:"Add State(s) to Queue__jki_lib_state_machine.vi"("State(s) in Front (\"\")"="UI: Initialize Status\nUI: Initialize Listbox\nUI: Initialize Render", "State(s) in (\"\")"=w636) -> ("States Out"=w635:string)  [unwired: 13 in]
          }
          frame "UI: Initialize Status" {
            # "Do not put any code in this frame.\n(It is a separator no-op. You can make a copy of this frame to create a new UI frame)"
            n257 = control-ref of="Status"() -> (w643:refnum<vi>)
            n258 = property class="Str"(reference=w643, error in=w640, "Text.FontName"="Consolas" ("Text.Font:Name"), "Text.FontSize"=u32 20 ("Text.Font:Size")) -> (error out=w641:errorcluster)  [unwired: 1 out]
            n259 = call <vilib>:"Add State(s) to Queue__jki_lib_state_machine.vi"("State(s) in (\"\")"=w646) -> ("States Out"=w647:string)  [unwired: 14 in]
          }
          frame "UI: Initialize Listbox" {
            w657 = TRUE ("Drag/Drop:Allow Dragging")
            # "Make listbox look like JKI Flat 2.0"
            # "Initialize the User Interface, here.\n(this is called automatically, by the Macro: Init)"
            n260 = Unbundle By Name(w652) -> ("MCLB"=w649:refnum<class "Selector.lvclass">)
            n261 = control-ref of="Patterns"() -> (w666:refnum<vi>)
            n262 = property on="Property Node" class="LstBox (strict)"(reference=w666, error in=w648, "Active Row"=-2 ("Active Row:Active Row Number"), "Allow Item Drag"=w657, "Allow Drop"=w657, "Top Row"=0) -> (reference out=w655:refnum<vi>, error out=w667:errorcluster, "Item Names"=w653:string[])
            n263 = Bundle By Name(cluster=w652, "Drag and Drop.Running"=w653) -> (w651:T20)
            n264 = property on="Property Node" class="LstBox (strict)"(reference=w655, error in=w667, "CellBG"=u32 16777215 ("Active Row:Cell Background Color"), "CellFontName"="Application Font" ("Font Name"), "CellFontSize"=u32 22 ("Size"), "CellFontColor"=u32 3947580 ("Color"), "SelColor"=u32 11908533 ("Active Row:Cell Background Color")) -> (error out=w660:errorcluster)  [unwired: 1 out]
            n265 = Bundle By Name(cluster=w651, "MCLB"=w649) -> (w650:T20)
            n266 = Merge Errors(w660, w648) -> (w656:errorcluster)
            n267 = call <vilib>:"Add State(s) to Queue__jki_lib_state_machine.vi"("State(s) in (\"\")"=w669) -> ("States Out"=w668:string)  [unwired: 14 in]
          }
          frame "UI: Initialize Render" {
            w676 = FALSE
            w677 = TRUE
            # "Make a JKI Flat UI 2.0 IMAQ control."
            # "Initialize the User Interface, here.\n(this is called automatically, by the Macro: Init)"
            n268 = control-ref of="Render"() -> (w670:refnum<vi>)
            n269 = property on="Property Node" class="ImageControl"(reference=w670, error in=w672, "Annulus Tool Button Visible"=w676, "Closed Freehand Tool Button Visible"=w676, "Ellipse Tool Button Visible"=w676, "Freehand Tool Button Visible"=w676, "Line Tool Button Visible"=w676, "Pan Tool Button Visible"=w677, "Point Tool Button Visible"=w677, "Polygon Tool Button Visible"=w676, "Polyline Tool Button Visible"=w676, "Rectangle Tool Button Visible"=w676, "Rotated Rectangle Tool Button Visible"=w676, "Selection Tool Button Visible"=w677, "Zoom Tool Button Visible"=w677, "Zoom to Fit Mode"=TRUE) -> (error out=w675:errorcluster)  [unwired: 1 out]
            n270 = Merge Errors(w675) -> (w673:errorcluster)
            n271 = call <vilib>:"Add State(s) to Queue__jki_lib_state_machine.vi"("State(s) in (\"\")"=w679) -> ("States Out"=w678:string)  [unwired: 14 in]
          }
          frame "UI: Status" {
            w682 = "\r\n"
            # "Do not put any code in this frame.\n(It is a separator no-op. You can make a copy of this frame to create a new UI frame)"
            n272 = Unbundle By Name(w694) -> ("Status"=w689:string)
            n273 = Format Date/Time String(time format string (%c)="%H:%M:%S --") -> (date/time string=w691:string)  [unwired: 2 in]
            n274 = Concatenate Strings(w691, "\t", w688, w682, w689) -> (w683:string)
            n275 = call <vilib>:"Delimited String to 1D String Array.vi"("delimiter"=w682, "delimited string"=w683) -> ("string array"=w687:string[])  [unwired: 9 in]
            n276 = Array Subset(array=w687, index=0, length=100) -> (w684:string[])
            n277 = call <vilib>:"1D String Array to Delimited String.vi"("delimiter"=w682, "string array"=w684) -> ("delimited string"=w681:string)  [unwired: 9 in]
            "Status" <- w681
            n278 = Bundle By Name(cluster=w694, "Status"=w681) -> (w693:T20)
            n279 = call <vilib>:"Add State(s) to Queue__jki_lib_state_machine.vi"("State(s) in (\"\")"=w696) -> ("States Out"=w697:string)  [unwired: 14 in]
          }
          frame "UI: Ready" {
            # "Do not put any code in this frame.\n(It is a separator no-op. You can make a copy of this frame to create a new UI frame)"
            n280 = Match True/False String(2:"FALSE" ("false string"), 3:"TRUE" ("true string"), 4:w700) -> (0:→"Ready?":bool)  [unwired: 1 out]
            n281 = call <vilib>:"Add State(s) to Queue__jki_lib_state_machine.vi"("State(s) in (\"\")"=w705) -> ("States Out"=w706:string)  [unwired: 14 in]
          }
          frame "UI: Update Time" {
            # "Do not put any code in this frame.\n(It is a separator no-op. You can make a copy of this frame to create a new UI frame)"
            n282 = call <vilib>:"Add State(s) to Queue__jki_lib_state_machine.vi"("State(s) in (\"\")"=w711) -> ("States Out"=w712:string)  [unwired: 14 in]
            "Estimated Time" <- w708
          }
          frame "UI: Cursor Set" {
            # "Argument"
            # "Set and Unset Cursor Busy.\n(Usage: \"UI: Cursor Set >> Busy|Idle\")"
            n283 = Unbundle By Name(w714) -> ("Core.Current VI Reference"=w716:refnum<vi>)
            n284 = call <userlib>:"Tick Count (ms)__ogtk.vi"("error in (no error)"=w715) -> ("error out"=w721:errorcluster, "millisecond timer value"=w717:u32)  [unwired: 9 in]
            n285 = case shown="\"Busy\"" w724 {
              tunnel: w721 -> [w728 w731]
              tunnel: [w727 w730] -> w720
              tunnel: w716 -> [w726 w729]
              frame "Idle", Default {
                n286 = call <vilib>:"Unset Busy.vi"("error in (no error)"=w728, "VI reference (current VI)"=w726) -> ("error out"=w727:errorcluster)  [unwired: 9 in]
              }
              frame "Busy" {
                n287 = call <vilib>:"Set Busy.vi"("error in (no error)"=w731, "VI reference (current VI)"=w729) -> ("error out"=w730:errorcluster)  [unwired: 8 in, 1 out]
              }
            }
            n288 = call <userlib>:"Tick Count (ms)__ogtk.vi"("error in (no error)"=w720) -> ("error out"=w719:errorcluster, "millisecond timer value"=w718:u32)  [unwired: 9 in]
            n289 = Subtract(x=w718, y=w717) -> ()  [unwired: 1 out]
            n290 = call <vilib>:"Add State(s) to Queue__jki_lib_state_machine.vi"("State(s) in (\"\")"=w723) -> ("States Out"=w725:string)  [unwired: 14 in]
          }
          frame "UI: Front Panel State" {
            # "Argument"
            # "Set Front Panel Open or Closed\n(Usage: \"UI: Front Panel State >> Open|Close\")"
            n291 = Unbundle By Name(w733) -> ("Core.Current VI Reference"=w736:refnum<vi>)
            n292 = case shown="\"Open\", Default" w735 {
              tunnel: w739 -> [w744 w756]
              tunnel: [w745 w757] -> w738
              tunnel: w736 -> [w742 w754]
              frame "Open", Default {
                n293 = property on="Property Node" class="VI"(reference=w742, error in=w744) -> (reference out=w741:refnum<vi>, error out=w743:errorcluster, "Front Panel.Open"=w740:bool)
                n294 = case shown="False" w740 {
                  tunnel: [w750 w751] -> w745
                  tunnel: w743 -> [w749 w751]
                  tunnel: w741 -> [w746 _]
                  frame False {
                    n295 = invoke on="Invoke Node" class="VI" method="FP.Open"(reference=w746, error in=w749, "Activate"=TRUE, "State"=T7."Standard") -> (error out=w750:errorcluster)  [unwired: 1 in, 4 out]
                  }
                  frame True {
                  }
                }
              }
              frame "Close" {
                n296 = property on="Property Node" class="VI"(reference=w754, error in=w756) -> (reference out=w753:refnum<vi>, error out=w755:errorcluster, "Front Panel.Open"=w752:bool)
                n297 = case shown="False" w752 {
                  tunnel: [w758 w761] -> w757
                  tunnel: w755 -> [w758 w760]
                  tunnel: w753 -> [_ w759]
                  frame False {
                  }
                  frame True {
                    n298 = invoke on="Invoke Node" class="VI" method="FP.Close"(reference=w759, error in=w760) -> (error out=w761:errorcluster)  [unwired: 1 in, 2 out]
                  }
                }
              }
            }
            n299 = call <vilib>:"Add State(s) to Queue__jki_lib_state_machine.vi"("State(s) in (\"\")"=w734) -> ("States Out"=w737:string)  [unwired: 14 in]
          }
          frame "UI: Overlay" {
            # "Do not put any code in this frame.\n(It is a separator no-op. You can make a copy of this frame to create a new UI frame)"
            n300 = Unbundle By Name(w764) -> ("Background Image"=w763:path, "Image Data Range"=w762:cluster{dbl, dbl})
            n301 = call "AFM_OverlayConfigurator.vi"("Error In"=w765, "Image Data Range (Main)"=w762, "Main Image (IBW)"=w763) -> ("Error Out"=w766:errorcluster)  [unwired: 8 in]
            n302 = call <vilib>:"Add State(s) to Queue__jki_lib_state_machine.vi"("State(s) in (\"\")"=w768) -> ("States Out"=w769:string)  [unwired: 14 in]
          }
          frame "UI: Enable Run" {
            # "Do not put any code in this frame.\n(It is a separator no-op. You can make a copy of this frame to create a new UI frame)"
            n303 = Match True/False String(2:"Disabled" ("false string"), 3:"Enabled" ("true string"), 4:w778) -> (0:w777:bool)  [unwired: 1 out]
            n304 = Select(t=T8."Enabled" ("Disabled"), s=w777, f=T8."Disabled and Grayed Out" ("Disabled")) -> (s? t:f=w776:T8)
            n305 = control-ref of="Run"() -> (w779:refnum<vi>)
            n306 = property class="Bool (strict)"(reference=w779, error in=w772, "DisabledEnum"=w776) -> (error out=w773:errorcluster)  [unwired: 1 out]
            n307 = call <vilib>:"Add State(s) to Queue__jki_lib_state_machine.vi"("State(s) in (\"\")"=w782) -> ("States Out"=w783:string)  [unwired: 14 in]
          }
          frame "UI: Inkscape Path" {
            # "Do not put any code in this frame.\n(It is a separator no-op. You can make a copy of this frame to create a new UI frame)"
            n308 = Unbundle By Name(w785) -> ("Inkscape File (.svg)"=w784:path)
            n309 = local write "Inkscape File (.svg)"(w784) -> ()
            n310 = call <vilib>:"Add State(s) to Queue__jki_lib_state_machine.vi"("State(s) in (\"\")"=w787) -> ("States Out"=w788:string)  [unwired: 14 in]
          }
          frame "UI: Background Path" {
            # "Do not put any code in this frame.\n(It is a separator no-op. You can make a copy of this frame to create a new UI frame)"
            n311 = Unbundle By Name(w795) -> ("Background Image"=w791:path)
            n312 = call <vilib>:"Get File Extension.vi"("error in (no error)"=w792, "file"=w791) -> ("error out"=w793:errorcluster, "filename without extension"=→"Image Filename":string, "dup file"=w790:path)  [unwired: 5 in, 2 out]
            n313 = local write "Background Image"(w790) -> ()
            n314 = call <vilib>:"Add State(s) to Queue__jki_lib_state_machine.vi"("State(s) in (\"\")"=w797) -> ("States Out"=w798:string)  [unwired: 14 in]
          }
          frame "UI: IMAQ Render" {
            w807 = T31 4 items=["Grayscale (U8)", "Grayscale (I16)", "Grayscale (SGL)", "Complex (CSG)", "RGB (U32)", "HSL (U32)", "RGB (U64)", "Grayscale (U16)"] ("Image Type")
            # "This removes the flickering when the imaq control was written to since it is by reference. So suppose you had a background image and data already in the control. Then the data gets updated and the user refreshes. It will rewrite the background image, then the new data. So you will have background with data, background, background with data. This creates a flickering effect. If you update the new image on a different reference, and then copy it to the display reference, it will be Image with old data, Image with new data. This does not flicker because there is not the image without data shown at any point."
            # "Do not put any code in this frame.\n(It is a separator no-op. You can make a copy of this frame to create a new UI frame)"
            n315 = call <userlib>:"Tick Count (ms)__ogtk.vi"("error in (no error)"=w808) -> ("error out"=w802:errorcluster, "millisecond timer value"=w799:u32)  [unwired: 9 in]
            n316 = Unbundle By Name(w812) -> ("IMAQ (Work)"=w804:T1)
            n317 = call "Imaq Create"("Image Name"="Render", "Image Type"=w807, "error in (no error)"=w802) -> ("New Image"=w811:T1, "error out"=w806:errorcluster)  [unwired: 2 in]
            n318 = call "IMAQ Copy"("error in (no error)"=w806, "Image Dst"=w811, "Image Src"=w804) -> ("error out"=w805:errorcluster, "Image Dst Out"=→"Render":T1)  [unwired: 3 in]
            n319 = call <userlib>:"Tick Count (ms)__ogtk.vi"("error in (no error)"=w805) -> ("error out"=w801:errorcluster, "millisecond timer value"=w800:u32)  [unwired: 9 in]
            n320 = Subtract(x=w800, y=w799) -> ()  [unwired: 1 out]
            n321 = call <vilib>:"Add State(s) to Queue__jki_lib_state_machine.vi"("State(s) in Front (\"\")"="UI: Status >> IMAQ Rendered" ("State(s) in Front (\"\")"), "State(s) in (\"\")"=w814) -> ("States Out"=w815:string)  [unwired: 13 in]
          }
          frame "UI: Autosave Render" {
            # "Do not put any code in this frame.\n(It is a separator no-op. You can make a copy of this frame to create a new UI frame)"
            n322 = Unbundle By Name(w821) -> ("IMAQ (Work)"=w820:T1, "Autosave Path"=w819:path)
            n323 = call "IMAQ Merge Overlay"("error in (no error)"=w817, "Image Src"=w820) -> ("error out"=w823:errorcluster, "Image Dst Out"=w822:T1)  [unwired: 8 in]
            n324 = call-poly "IMAQ Write File 2"("error in (no error)"=w823, "Image Quality"=u32 512, "File Path"=w819, "Image"=w822) -> ("error out"=w818:errorcluster)  [unwired: 6 in, 1 out]
            n325 = call <vilib>:"Add State(s) to Queue__jki_lib_state_machine.vi"("State(s) in (\"\")"=w825) -> ("States Out"=w826:string)  [unwired: 14 in]
          }
          frame "UI: Autosave Render Path" {
            # "Do not put any code in this frame.\n(It is a separator no-op. You can make a copy of this frame to create a new UI frame)"
            n326 = Unbundle By Name(w830) -> ("Autosave Path"=w828:path, "Autosave?"=w827:bool)
            n327 = local write "Autosave?"(w827) -> ()
            n328 = local write "Autosave Path"(w828) -> ()
            n329 = call <vilib>:"Add State(s) to Queue__jki_lib_state_machine.vi"("State(s) in (\"\")"=w832) -> ("States Out"=w833:string)  [unwired: 14 in]
          }
          frame "UI: Update Subpanel" {
            # "Subpanel is updated to reflect pattern's type."
            n330 = control-ref of="Patterns"() -> (w851:refnum<vi>)
            n331 = Unbundle By Name(w855) -> ("VI Refs"=w835:refnum<vi>[])
            n332 = property class="LstBox (strict)"(reference=w851, error in=w834) -> (error out=w839:errorcluster, "Item Names"=w848:string[], "Value"=w845:i32)  [unwired: 1 out]
            n333 = control-ref of="Properties"() -> (w846:refnum<vi>)
            n334 = Index Array(array=w848, index=w845) -> (element=w840:string)
            n335 = Search/Split String(string=w840, offset (0)=1) -> (substring before match=w847:string)  [unwired: 1 in, 2 out]
            n336 = call <vilib>:"Build State String with Arguments__JKI_lib_State_Machine.vi"("Arguments (\"\")"=w840, "State"="Database: Set Active") -> ("State with Arguments"=w849:string)  [unwired: 4 in]
            n337 = case shown="\"d\"" w847 {
              tunnel: [2 3 0 1] -> w852
              frame "f", Default {
              }
              frame "d" {
              }
              frame "p" {
              }
              frame "r" {
              }
            }
            n338 = property class="SubPnl"(reference=w846, error in=w839) -> (reference out=w841:refnum<vi>, error out=w842:errorcluster, "InsertedVI"=w837:refnum<vi>)
            n339 = Index Array(array=w835, index=w852) -> (element=w838:refnum<vi>)
            n340 = Equal?(x=w838, y=w837) -> (x = y?=w843:bool)
            n341 = case shown="False" w843 {
              tunnel: w842 -> [w861 w863]
              tunnel: [w860 w863] -> w836
              tunnel: w838 -> [w859 _]
              tunnel: w841 -> [w858 _]
              frame False {
                n342 = invoke on="Invoke Node" class="SubPnl" method="Remove VI"(reference=w858, error in=w861) -> (reference out=w857:refnum<vi>, error out=w862:errorcluster)  [unwired: 1 in, 1 out]
                n343 = invoke on="Invoke Node" class="SubPnl" method="Insert VI"(reference=w857, error in=w862, "VI Ref"=w859) -> (error out=w860:errorcluster)  [unwired: 1 in, 3 out]
              }
              frame True {
              }
            }
            n344 = call <vilib>:"Add State(s) to Queue__jki_lib_state_machine.vi"("State(s) in Front (\"\")"=w849, "State(s) in (\"\")"=w854) -> ("States Out"=w856:string)  [unwired: 13 in]
          }
          frame "UI: Update AFM Ring" {
            # "populate AFM Type ring"
            # "Do not put any code in this frame.\n(It is a separator no-op. You can make a copy of this frame to create a new UI frame)"
            n345 = Select(t=string[] ["Asylum"], s=TRUE, f=string[] ["Cypher", "MFP3D", "MFP3D_Lucy", "Simulation"] ("folder names")) -> (s? t:f=w868:string[])
            n346 = property on="AFM Type" class="Ring (strict)"(error in=w870, "Strings []"=w868) -> (error out=w869:errorcluster)  [unwired: 1 in, 1 out]
            n347 = call <vilib>:"Add State(s) to Queue__jki_lib_state_machine.vi"("State(s) in (\"\")"=w876) -> ("States Out"=w877:string)  [unwired: 14 in]
          }
          frame "---------- Macro ----------" {
            # "Do not put any code in this frame.\n(It is a separator no-op. You can make a copy of this frame to create a new Macro frame)"
            n348 = call <vilib>:"Add State(s) to Queue__jki_lib_state_machine.vi"("State(s) in (\"\")"=w880) -> ("States Out"=w881:string)  [unwired: 14 in]
          }
          frame "Macro: Start SMOs" {
            # "Do not put any code in this frame.\n(It is a separator no-op. You can make a copy of this frame to create a new Macro frame)"
            n349 = call <vilib>:"Add State(s) to Queue__jki_lib_state_machine.vi"("State(s) in Front (\"\")"="Parser: Start\nDatabase: Start\nTooler: Start\nDriver: Init Manager", "State(s) in (\"\")"=w886) -> ("States Out"=w887:string)  [unwired: 13 in]
          }
          frame "Macro: Start Driver" {
            # "Do not put any code in this frame.\n(It is a separator no-op. You can make a copy of this frame to create a new Macro frame)"
            n350 = call <vilib>:"Add State(s) to Queue__jki_lib_state_machine.vi"("State(s) in Front (\"\")"="Driver: Init Drivers\nDriver: Set Active\nDriver: Insert Into Subpanel >> 0", "State(s) in (\"\")"=w892) -> ("States Out"=w893:string)  [unwired: 13 in]
          }
          frame "Macro: Reorder" {
            # "Do not put any code in this frame.\n(It is a separator no-op. You can make a copy of this frame to create a new Macro frame)"
            n351 = call <vilib>:"Add State(s) to Queue__jki_lib_state_machine.vi"("State(s) in (\"\")"=w897) -> ("States Out"=w898:string)  [unwired: 14 in]
          }
          frame "Macro: Litho Data" {
            # "Do not put any code in this frame.\n(It is a separator no-op. You can make a copy of this frame to create a new Macro frame)"
            n352 = call <vilib>:"Add State(s) to Queue__jki_lib_state_machine.vi"("State(s) in Front (\"\")"="Litho: Update Information\nListbox: Compare Values\nListbox: Reorder Data\nLitho: Order Data\nDriver: Litho Data\nLitho: Refresh Render" ("State(s) in Front (\"\")"), "State(s) in (\"\")"=w903) -> ("States Out"=w904:string)  [unwired: 13 in]
          }
          frame "Macro: Properties Updated" {
            # "Do not put any code in this frame.\n(It is a separator no-op. You can make a copy of this frame to create a new Macro frame)"
            n353 = call <vilib>:"Add State(s) to Queue__jki_lib_state_machine.vi"("State(s) in Front (\"\")"="//Idle\nUI: Status >> Object Properties Updated\nUI: Ready >> FALSE\nMCLB: Symbols\nMacro: Litho Data\nUI: IMAQ Render\nUI: Ready >> TRUE", "State(s) in (\"\")"=w909) -> ("States Out"=w910:string)  [unwired: 13 in]
          }
          frame "Macro: Send Driver" {
            # "Information that we want to send to the driver all at once. Ie background image and lithography data"
            n354 = call <vilib>:"Add State(s) to Queue__jki_lib_state_machine.vi"("State(s) in Front (\"\")"="Driver: Background Image\nDriver: Litho Data", "State(s) in (\"\")"=w915) -> ("States Out"=w916:string)  [unwired: 13 in]
          }
          frame "Macro: Refresh" {
            # "Do not put any code in this frame.\n(It is a separator no-op. You can make a copy of this frame to create a new Macro frame)"
            n355 = call <vilib>:"Add State(s) to Queue__jki_lib_state_machine.vi"("State(s) in Front (\"\")"="Litho: Load SVG\nParser: Parse SVG\nDatabase: Refresh Sync\nLitho: Load Background\nLitho: Display Background\nMacro: Litho Data\nUI: IMAQ Render", "State(s) in (\"\")"=w921) -> ("States Out"=w922:string)  [unwired: 13 in]
          }
          frame "Macro: Initialize" {
            w926 = FALSE  # debug?
            w928 = "Data: Initialize\nInitialize Core Data\nConfiguration: Initialize\nConfiguration: Read\nEvents: Register\n\nUI: Initialize\nUI: Front Panel State >> Open\n\nData: Set Root Path"  # macro for debugging
            # "On start up:\nData Initialize\nInitialize core data\nPrep the UI\nRead configuration\nStart Subsystems\nRegister for events\nInitialize the UI\nRun the editing VI subpanels\nStart up the AFM driver\nLoad up the SVG\nParse the SVG \nInitialize the database\nRead and display the background image\nTool the data based on default settings\nUpdate and populate the listbox\nUse the listbox to reorder the data\nSend the data to the driver\nRender the overlay on the svg\nCopy the overlay to the IMAQ display"
            # "Initialization Macro\n(This is called once, when the VI starts)"
            n356 = Select(t=w928, s=w926, f="Data: Initialize\nInitialize Core Data\nUI: Ready >> FALSE\nUI: Cursor Set >> Busy\nConfiguration: Initialize\nConfiguration: Read\nMacro: Start SMOs\nEvents: Register\nUI: Initialize\nUI: Enable Run >> Enabled\nUI: Front Panel State >> Open\nData: Set Root Path\nData: Run Edit VIs\nUI: Update AFM Ring\nUI: Update Subpanel\nMacro: Start Driver\nMacro: Refresh\nMacro: Send Driver\nUI: Ready >> TRUE\nUI: Cursor Set >> Idle") -> (s? t:f=w927:string)
            n357 = call <vilib>:"Add State(s) to Queue__jki_lib_state_machine.vi"("State(s) in Front (\"\")"=w927, "State(s) in (\"\")"=w929) -> ("States Out"=w931:string)  [unwired: 13 in]
          }
          frame "Macro: Exit" {
            # "Why is database so far at the end??"
            # "Exit Macro\n(This is called once, when the VI exits)"
            n358 = Unbundle By Name(w935) -> ("Core.Close Panel on Exit?"=w941:bool)
            n359 = Select(t="UI: Front Panel State >> Close", s=w941, f="" ("Empty String Constant")) -> (s? t:f=w938:string)
            n360 = call <vilib>:"Add State(s) to Queue__jki_lib_state_machine.vi"("State(s) in (\"\")"=w938, "State(s) at Back (\"\")"="UI: Enable Run >> Enabled \\\\makes it easier when editing\nParser: Stop\nTooler: Stop\nDriver: Stop Manager\nConfiguration: Write\nData: Cleanup\nEvents: Unregister\nDatabase: Stop\nExit") -> ("States Out"=w936:string)  [unwired: 13 in]
            n361 = call <vilib>:"Add State(s) to Queue__jki_lib_state_machine.vi"("State(s) in Front (\"\")"=w936, "State(s) in (\"\")"=w934) -> ("States Out"=w942:string)  [unwired: 13 in]
          }
          frame "---------- Litho ----------" {
            # "Template Separator\n(You can make a copy of, or modify, this frame)"
            n362 = call <vilib>:"Add State(s) to Queue__jki_lib_state_machine.vi"("State(s) in (\"\")"=w946) -> ("States Out"=w947:string)  [unwired: 14 in]
          }
          frame "Litho: Load SVG" {
            # "Load SVG\nParses the SVG and stores the data obtained from it."
            n363 = Unbundle By Name(w964) -> ("Inkscape File (.svg)"=w961:path)
            n364 = call "CheckFileConformity.vi"("error in (no error)"=w962, "File Data"=T9 {"Pattern"="svg", "Pattern Label"="Scalable Vector Graphics", "Prompt"="Choose an SVG file"}, "Path In"=w961) -> ("error out"=w959:errorcluster, "No File"=w955:bool, "Path Out"=w960:path, "Asked to Change?"=w949:bool)  [unwired: 5 in]
            n365 = case shown="False" w955 {
              tunnel: w960 -> [w969 _]
              tunnel: w959 -> [w968 w972]
              tunnel: [w968 w974] -> w958
              tunnel: [w969 w973] -> w957
              frame False {
              }
              frame True {
                n366 = call "Display Message to User"("error in (no error)"=w972, "Message"="No Valid File Selected. Using Default.") -> ("error out"=w971:errorcluster)  [unwired: 8 in, 1 out]
                n367 = call "GenerateDefaultSVGFile.vi"("error in (no error)"=w971) -> ("error out"=w974:errorcluster, "Path"=w973:path)  [unwired: 9 in]
              }
            }
            n368 = Select(t="", s=w949, f="Configuration: Write") -> (s? t:f=w952:string)
            n369 = call <vilib>:"Add State(s) to Queue__jki_lib_state_machine.vi"("State(s) in Front (\"\")"="UI: Inkscape Path", "State(s) in (\"\")"=w952) -> ("States Out"=w950:string)  [unwired: 13 in]
            n370 = Bundle By Name(cluster=w964, "Inkscape File (.svg)"=w957) -> (w963:T20)
            n371 = call <vilib>:"Add State(s) to Queue__jki_lib_state_machine.vi"("State(s) in Front (\"\")"=w950, "State(s) in (\"\")"=w966) -> ("States Out"=w967:string)  [unwired: 13 in]
          }
          frame "Litho: Load Background" {
            # "Load Background\nLoads the background file into the images."
            n372 = Unbundle By Name(w989) -> ("Background Image"=w988:path)
            n373 = call "CheckFileConformity.vi"("error in (no error)"=w987, "File Data"=T9 {"Pattern"="ibw", "Pattern Label"="Igor Binary Wave", "Prompt"="Choose an IBW file"}, "Path In"=w988) -> ("error out"=w983:errorcluster, "No File"=w975:bool, "Path Out"=w985:path, "Asked to Change?"=w976:bool)  [unwired: 5 in]
            n374 = case shown="True" w975 {
              tunnel: w983 -> [w994 w997]
              tunnel: w985 -> [w995 _]
              tunnel: [w995 w999] -> w984
              tunnel: [w994 w1000] -> w982
              frame False {
              }
              frame True {
                n375 = call "Display Message to User3"("error in (no error)"=w997, "Message"="No Valid File Selected. Using Default.") -> ("error out"=w996:errorcluster)  [unwired: 8 in, 1 out]
                n376 = call "GenerateDefaultIBWFile.vi"("error in (no error)"=w996) -> ("error out"=w1000:errorcluster, "Path"=w999:path)  [unwired: 9 in]
              }
            }
            n377 = Select(t="", s=w976, f="Configuration: Write") -> (s? t:f=w979:string)
            n378 = Bundle By Name(cluster=w989, "Background Image"=w984) -> (w990:T20)
            n379 = call <vilib>:"Add State(s) to Queue__jki_lib_state_machine.vi"("State(s) in Front (\"\")"="UI: Background Path", "State(s) in (\"\")"=w979) -> ("States Out"=w977:string)  [unwired: 13 in]
            n380 = call <vilib>:"Add State(s) to Queue__jki_lib_state_machine.vi"("State(s) in Front (\"\")"=w977, "State(s) in (\"\")"=w992) -> ("States Out"=w993:string)  [unwired: 13 in]
          }
          frame "Litho: Display Background" {
            # "Added logic so user cannot select a page/image that doesnt exist"
            # "Displays the background from a file"
            n381 = Unbundle By Name(w1018) -> ("Background Image"=w1017:path, "Inkscape File (.svg)"=w1008:path)
            n382 = Unbundle("Image Data Range") -> (w1020:dbl, w1019:dbl)
            n383 = local read "Page"() -> (w1016:u32)
            n384 = Max & Min(x=w1020, y=w1019) -> (max(x,y)=w1003:dbl, min(x,y)=w1002:dbl)
            n385 = call "Background.vi"("Image data max"=w1003, "Image data min"=w1002, "error in (no error)"=w1021, "Resolution"=1024, "Page"=w1016, "Image File Path"=w1017) -> ("error out"=w1010:errorcluster, "Max Pages"=w1005:i32, "Corrected Page"=w1004:i32, "Background out"=w1007:T1)  [unwired: 2 in]
            n386 = control-ref of="Page"() -> (w1015:refnum<vi>)
            n387 = call "SaveBackground.vi"("error in (no error)"=w1010, "Path"=w1008, "Background In"=w1007) -> ("error out"=w1009:errorcluster, "Background Out"=w1006:T1)  [unwired: 7 in]
            n388 = property class="DigNum (strict)"(reference=w1015, error in=w1009, "Value"=w1004, "Maximum"=w1005) -> (error out=w1014:errorcluster)  [unwired: 1 out]
            n389 = Bundle(w1003, w1002) -> (w1001:cluster{dbl, dbl})  [unwired: 1 in]
            n390 = Bundle By Name(cluster=w1018, "Image Data Range"=w1001, "IMAQ (Work)"=w1006) -> (w1022:T20)
            n391 = call <vilib>:"Add State(s) to Queue__jki_lib_state_machine.vi"("State(s) in (\"\")"=w1023) -> ("States Out"=w1024:string)  [unwired: 14 in]
          }
          frame "Litho: Update Information" {
            # "Update the lithography data (toolpath)\nUses the parsing data and the properties of each pattern to generate the lithography data."
            n392 = call <vilib>:"Add State(s) to Queue__jki_lib_state_machine.vi"("State(s) in Front (\"\")"="Tooler: Objects\nUI: Status >> Settings applied to objects" ("State(s) in Front (\"\")"), "State(s) in (\"\")"=w1027) -> ("States Out"=w1029:string)  [unwired: 13 in]
          }
          frame "Litho: Order Data" {
            n393 = disable-structure shown="Enabled" {
              disable-tunnel: [w1056 w1060] -> w1038
              disable-tunnel: w1037 -> [w1055 w1060]
              disable-tunnel: [w1048 _] -> w1035
              disable-tunnel: w1034 -> [w1046 w1061]
              disable-tunnel: [w1044 w1061] -> w1033
              disable-tunnel: [w1041 _] -> _
              disable-tunnel: [w1040 w1059] -> w1032
              disable-tunnel: w1031 -> [w1040 w1059]
              frame Disabled {
                # "Order the Patterns\nUses the ordering data to fix lithography data."
                n394 = call <userlib>:"Tick Count (ms)__ogtk.vi"("error in (no error)"=w1046) -> ("error out"=w1047:errorcluster, "millisecond timer value"=w1043:u32)  [unwired: 9 in]
                n395 = Unbundle By Name(w1055) -> ("Lithography Data"=w1057:T27)
                n396 = control-ref of="Patterns"() -> (w1054:refnum<vi>)
                n397 = call "Order Patterns.vi"("error in (no error)"=w1047, "Lithography Data"=w1057, "ListBox Reference in"=w1054) -> ("error out"=w1045:errorcluster, "Order Unchanged"=w1049:bool, "Ordered Lithography Data"=w1058:T27)  [unwired: 6 in]
                n398 = Bundle By Name(cluster=w1055, "Lithography Data"=w1058) -> (w1056:T20)
                n399 = call <userlib>:"Tick Count (ms)__ogtk.vi"("error in (no error)"=w1045) -> ("error out"=w1044:errorcluster, "millisecond timer value"=w1042:u32)  [unwired: 9 in]
                n400 = Subtract(x=w1042, y=w1043) -> (x-y=w1041:u32)
                n401 = Select(t="Unchanged Object Order Applied to Data", s=w1049, f="New Object Order Applied to Data" ("Arguments (\"\")")) -> (s? t:f=w1052:string)
                n402 = call <vilib>:"Build State String with Arguments__JKI_lib_State_Machine.vi"("Arguments (\"\")"=w1052, "State"="UI: Status") -> ("State with Arguments"=w1048:string)  [unwired: 4 in]
              }
              frame Enabled {
              }
            }
            n403 = call <vilib>:"Add State(s) to Queue__jki_lib_state_machine.vi"("State(s) in Front (\"\")"=w1035, "State(s) in (\"\")"=w1032) -> ("States Out"=w1039:string)  [unwired: 13 in]
          }
          frame "Litho: Refresh Render" {
            # "Update the images\nUses the lithography data to update the images."
            n404 = Unbundle By Name(w1073) -> ("Lithography Data"=w1079:T27, "IMAQ (Work)"=w1076:T1, "Hide Labels"=w1071:bool, "Autosave?"=w1070:bool)
            n405 = call "Image Generator.vi"("Coerce"=TRUE, "Hide Labels"=w1071, "Lithography Data"=w1079, "error in (no error)"=w1063, "Resolution"=1024, "Image Reference In"=w1076) -> ("error out"=w1062:errorcluster, "Image Reference Out"=w1075:T1)  [unwired: 4 in]
            n406 = Bundle By Name(cluster=w1073, "IMAQ (Work)"=w1075) -> (w1074:T20)
            n407 = Select(t="UI: Autosave Render", s=w1070, f="") -> (s? t:f=w1065:string)
            n408 = call <vilib>:"Add State(s) to Queue__jki_lib_state_machine.vi"("State(s) in Front (\"\")"="UI: Status >> Render Refreshed" ("State(s) in (\"\")"), "State(s) in (\"\")"=w1065) -> ("States Out"=w1067:string)  [unwired: 13 in]
            n409 = call <vilib>:"Add State(s) to Queue__jki_lib_state_machine.vi"("State(s) in Front (\"\")"=w1067, "State(s) in (\"\")"=w1078) -> ("States Out"=w1080:string)  [unwired: 13 in]
          }
          frame "---------- Listbox ----------" {
            # "Template Separator\n(You can make a copy of, or modify, this frame)"
            n410 = call <vilib>:"Add State(s) to Queue__jki_lib_state_machine.vi"("State(s) in (\"\")"=w1082) -> ("States Out"=w1084:string)  [unwired: 14 in]
          }
          frame "Listbox: Compare Values" {
            # "If working is what is al"
            # "Do they have the same"
            # "This should be the only place that we set the running data."
            # "Template Separator\n(You can make a copy of, or modify, this frame)"
            n411 = Unbundle By Name(w1094) -> ("Drag and Drop.Running"=w1092:string[], "Drag and Drop.Working"=w1091:string[])
            n412 = Sort 1D Array(array=w1092) -> (sorted array=w1095:string[])
            n413 = Sort 1D Array(array=w1091) -> (sorted array=w1096:string[])
            n414 = Equal?(x=w1095, y=w1096) -> (x = y?=w1097:bool)
            n415 = case shown="False" w1097 {
              tunnel: w1092 -> [w1102 w1117]
              tunnel: w1091 -> [w1106 _]
              tunnel: [w1107 w1117] -> w1086
              frame False {
                n416 = for {
                  tunnel: w1102 -> [w1115]
                  tunnel: w1106 -> [w1112] mode=indexing
                  tunnel: [w1112] -> w1108 mode=indexing if=w1116
                  tunnel: [w1114] -> w1105 mode=indexing if=w1113
                  n417 = Search 1D Array(1D array=w1115, element=w1112) -> (index of element=w1114:i32)  [unwired: 1 in]
                  n418 = Greater Or Equal To 0?(x=w1114) -> (x >= 0?=w1113:bool)
                  n419 = Not(x=w1113) -> (.not. x?=w1116:bool)
                }
                n420 = Sort 1D Array(array=w1105) -> (sorted array=w1104:i32[])
                n421 = for {
                  tunnel: w1102 -> [w1111]
                  tunnel: w1104 -> [w1110] mode=indexing
                  tunnel: [w1109] -> w1103 mode=indexing
                  n422 = Index Array(array=w1111, index=w1110) -> (element=w1109:string)
                }
                n423 = Build Array (concatenate)(w1103, w1108) -> (w1107:string[])
              }
              frame True {
              }
            }
            n424 = Equal?(x=w1092, y=w1086) -> (x = y?=w1090:bool)
            n425 = Bundle By Name(cluster=w1094, "Drag and Drop.Running"=w1086) -> (w1093:T20)
            n426 = Select(t="", s=w1090, f="Listbox: Populate") -> (s? t:f=w1087:string)
            n427 = call <vilib>:"Add State(s) to Queue__jki_lib_state_machine.vi"("State(s) in Front (\"\")"=w1087, "State(s) in (\"\")"=w1099) -> ("States Out"=w1100:string)  [unwired: 13 in]
          }
          frame "Listbox: Populate" {
            # "Template Separator\n(You can make a copy of, or modify, this frame)"
            n428 = Unbundle By Name(w1125) -> ("Drag and Drop.Running"=w1121:string[])
            n429 = control-ref of="Patterns"() -> (w1124:refnum<vi>)
            n430 = property class="LstBox (strict)"(reference=w1124, error in=w1120, "Item Names"=w1121, "Value"=0) -> (error out=w1118:errorcluster)  [unwired: 1 out]
            n431 = Merge Errors(w1118) -> (w1119:errorcluster)
            n432 = call <vilib>:"Add State(s) to Queue__jki_lib_state_machine.vi"("State(s) in Front (\"\")"="UI: Update Subpanel", "State(s) in (\"\")"=w1127) -> ("States Out"=w1128:string)  [unwired: 13 in]
          }
          frame "Listbox: Reorder Data" {
            # "Template Separator\n(You can make a copy of, or modify, this frame)"
            n433 = Unbundle By Name(w1133) -> ("Drag and Drop.Running"=w1137:string[], "Lithography Data"=w1136:T27)
            n434 = for {
              shift-right: [w1154] -> w1131
              shift-left: w1137 -> [w1154]
              tunnel: w1136 -> [w1152] mode=indexing
              tunnel: [w1153] -> w1129 mode=indexing
              tunnel: [w1152] -> w1135 mode=indexing
              n435 = Unbundle By Name(w1152) -> ("Name"=w1153:string)
            }
            n436 = Equal?(x=w1131, y=w1129) -> (x = y?=w1130:bool)
            n437 = case shown="False" w1130 {
              tunnel: w1135 -> [w1145 w1151]
              tunnel: [w1144 w1151] -> w1132
              tunnel: w1131 -> [w1143 _]
              tunnel: w1129 -> [w1142 _]
              frame False {
                # "reorder items in lithography"
                n438 = for {
                  tunnel: w1142 -> [w1150]
                  tunnel: w1143 -> [w1149] mode=indexing
                  tunnel: w1145 -> [w1148]
                  tunnel: [w1146] -> w1144 mode=indexing
                  n439 = Search 1D Array(1D array=w1150, element=w1149) -> (index of element=w1147:i32)  [unwired: 1 in]
                  n440 = Index Array(array=w1148, index=w1147) -> (element=w1146:T32)
                }
              }
              frame True {
                # "Order is already correct"
              }
            }
            n441 = Bundle By Name(cluster=w1133, "Lithography Data"=w1132) -> (w1134:T20)
            n442 = call <vilib>:"Add State(s) to Queue__jki_lib_state_machine.vi"("State(s) in (\"\")"=w1139) -> ("States Out"=w1140:string)  [unwired: 14 in]
          }
          frame "---------- MCLB ----------" {
            # "Multicolumn Listbox\n(You can make a copy of, or modify, this frame)"
            n443 = Unbundle By Name(w1156) -> ("MCLB"=w1155:refnum<class "Selector.lvclass">)
            n444 = Bundle By Name(cluster=w1156, "MCLB"=w1155) -> (w1157:T20)
            n445 = call <vilib>:"Add State(s) to Queue__jki_lib_state_machine.vi"("State(s) in (\"\")"=w1159) -> ("States Out"=w1160:string)  [unwired: 14 in]
          }
          frame "MCLB: Symbols" {
            # "Multicolumn Listbox\n(You can make a copy of, or modify, this frame)"
            n446 = Unbundle By Name(w1164) -> ("MCLB"=w1162:refnum<class "Selector.lvclass">)
            n447 = Bundle By Name(cluster=w1164, "MCLB"=w1162) -> (w1165:T20)
            n448 = call <vilib>:"Add State(s) to Queue__jki_lib_state_machine.vi"("State(s) in (\"\")"=w1167) -> ("States Out"=w1168:string)  [unwired: 14 in]
          }
          frame "MCLB: Reorder" {
            # "Multicolumn Listbox\n(You can make a copy of, or modify, this frame)"
            n449 = Unbundle By Name(w1178) -> ("MCLB"=w1176:refnum<class "Selector.lvclass">, "Item Names"=w1170:string[][])
            n450 = call-dynamic "Read Items.vi"("Selector in"=w1176) -> ("Items"=w1175:T33, "Selector out"=w1174:refnum<class "Selector.lvclass">)  [unwired: 8 in, 1 out]
            n451 = Index Array(array=w1170, index (col)=0 ("disabled index (col)")) -> (element=w1169:string[])  [unwired: 1 in]
            n452 = call "Items to Names.vi"("Items"=w1175) -> ("Names"=w1177:string[])  [unwired: 6 in]
            n453 = for {
              tunnel: w1175 -> [w1186]
              tunnel: w1177 -> [w1188]
              tunnel: w1169 -> [w1187] mode=indexing
              tunnel: [w1184] -> w1172 mode=indexing
              n454 = Search 1D Array(1D array=w1188, element=w1187) -> (index of element=w1185:i32)  [unwired: 1 in]
              n455 = Index Array(array=w1186, index=w1185) -> (element=w1184:T10)
            }
            n456 = call-dynamic "Write Items.vi"("Items"=w1172, "Selector in"=w1174) -> ("Selector out"=w1173:refnum<class "Selector.lvclass">)  [unwired: 8 in, 1 out]
            n457 = Bundle By Name(cluster=w1178, "MCLB"=w1173) -> (w1179:T20)
            n458 = call <vilib>:"Add State(s) to Queue__jki_lib_state_machine.vi"("State(s) in (\"\")"=w1181) -> ("States Out"=w1182:string)  [unwired: 14 in]
          }
          frame "MCLB: SCM Selection" {
            # "Multicolumn Listbox\n(You can make a copy of, or modify, this frame)"
            n459 = Unbundle By Name(w1192) -> ("Database"=w1191:refnum<class "Setting Database.lvclass">, "MCLB"=w1190:refnum<class "Selector.lvclass">)  [unwired: 1 out]
            n460 = Bundle By Name(cluster=w1192, "Database"=w1191, "MCLB"=w1190) -> (w1193:T20)
            n461 = call <vilib>:"Add State(s) to Queue__jki_lib_state_machine.vi"("State(s) in (\"\")"=w1195) -> ("States Out"=w1196:string)  [unwired: 14 in]
          }
          frame "MCLB: Populate New" {
            # "Multicolumn Listbox\n(You can make a copy of, or modify, this frame)"
            n462 = Unbundle By Name(w1198) -> ("MCLB"=w1197:refnum<class "Selector.lvclass">)
            n463 = Bundle By Name(cluster=w1198, "MCLB"=w1197) -> (w1199:T20)
            n464 = call <vilib>:"Add State(s) to Queue__jki_lib_state_machine.vi"("State(s) in (\"\")"=w1201) -> ("States Out"=w1202:string)  [unwired: 14 in]
          }
          frame "MCLB: Generate Names" {
            # "Multicolumn Listbox\n(You can make a copy of, or modify, this frame)"
            n465 = Unbundle By Name(w1221) -> ("MCLB"=w1212:refnum<class "Selector.lvclass">, "Tooler"=w1220:refnum<class "Tool Data.lvclass">, "IDs.paths"=w1219:string[], "IDs.funnels"=w1218:string[], "IDs.rects"=w1217:string[], "IDs.dots"=w1216:string[])
            n466 = Array Size(array=w1218) -> (size(s)=w1206:i32)
            n467 = Array Size(array=w1219) -> (size(s)=w1207:i32)
            n468 = Array Size(array=w1217) -> (size(s)=w1205:i32)
            n469 = Array Size(array=w1216) -> (size(s)=w1204:i32)
            n470 = Build Array(w1207, w1206, w1205, w1204) -> (w1215:i32[])
            n471 = for {
              tunnel: w1215 -> [w1227] mode=indexing
              tunnel: string[] ["p", "f", "r", "d"] -> [w1229] mode=indexing
              tunnel: [w1228] -> w1209 mode=concatenating
              n472 = for {
                N: w1227 -> [_]
                tunnel: w1229 -> [w1234]
                tunnel: [w1230] -> w1228 mode=indexing
                i -> [w1235]
                n473 = Number To Decimal String(number=w1235) -> (decimal integer string=w1233:string)  [unwired: 1 in]
                n474 = Concatenate Strings(w1234, w1233) -> (w1231:string)
                n475 = Bundle By Name(cluster=T10 {"Name"="", "Group"="", "Enabled"=FALSE} ("element"), "Name"=w1231) -> (w1230:T10)
              }
            }
            n476 = call-dynamic "Read Reference.vi"("Selector in"=w1212) -> ("Reference"=w1210:refnum<vi>, "Selector out"=w1211:refnum<class "Selector.lvclass">)  [unwired: 8 in, 1 out]
            n477 = call "Items to MCLB Item Names.vi"("Items"=w1209) -> ("Item Names"=w1208:string[][])  [unwired: 6 in]
            n478 = call-dynamic "Write Items.vi"("Items"=w1209, "Selector in"=w1211) -> ("Selector out"=w1213:refnum<class "Selector.lvclass">)  [unwired: 8 in, 1 out]
            n479 = property class="MCListbox"(reference=w1210, "ItemNames"=w1208) -> ()  [unwired: 1 in, 2 out]
            n480 = Bundle By Name(cluster=w1221, "MCLB"=w1213, "Tooler"=w1220) -> (w1222:T20)
            n481 = call <vilib>:"Add State(s) to Queue__jki_lib_state_machine.vi"("State(s) in (\"\")"=w1224) -> ("States Out"=w1225:string)  [unwired: 14 in]
          }
          frame "---------- Configuration ----------" {
            # "Template Separator\n(You can make a copy of, or modify, this frame)"
            n482 = Unbundle By Name(w1237) -> ("Background Image"=w1236:path)
            n483 = Bundle By Name(cluster=w1237, "Background Image"=w1236) -> (w1238:T20)
            n484 = call <vilib>:"Add State(s) to Queue__jki_lib_state_machine.vi"("State(s) in (\"\")"=w1240) -> ("States Out"=w1241:string)  [unwired: 14 in]
          }
          frame "Configuration: Write" {
            # "Write new information to the configuration file for next time we use program"
            n485 = Unbundle By Name(w1254) -> ("Config"=w1243:refnum<class "Configuration.lvclass">, "Inkscape File (.svg)"=w1252:path, "Background Image"=w1251:path, "Autosave Path"=w1250:path, "Autosave?"=w1249:bool)
            n486 = Bundle(cluster=T11 {"Inkscape Path"=path "", "Background Path"=path "", "Autosave Render Path"=path "", "Autosave Render"=FALSE, "Hide Labels"=FALSE, "Normal Render Path"=path "", "Overwrite"=FALSE} ("Configuration Data"), "Inkscape Path"=w1252, "Background Path"=w1251, "Autosave Render Path"=w1250, "Autosave Render"=w1249) -> (w1244:T11)  [unwired: 3 in]
            n487 = call <userlib>:"Write Configuration.vi"("error in (no error)"=w1246, "Variant"=w1244, "Configuration in"=w1243) -> ("error out"=w1245:errorcluster, "Configuration out"=w1247:refnum<class "Configuration.lvclass">)  [unwired: 7 in]
            n488 = Bundle By Name(cluster=w1254, "Config"=w1247) -> (w1255:T20)
            n489 = call <vilib>:"Add State(s) to Queue__jki_lib_state_machine.vi"("State(s) in Front (\"\")"="UI: Status >> Configuration Written" ("State(s) in Front (\"\")"), "State(s) in (\"\")"=w1257) -> ("States Out"=w1258:string)  [unwired: 13 in]
          }
          frame "Configuration: Read" {
            w1267 = T11 {"Inkscape Path"=path "", "Background Path"=path "", "Autosave Render Path"=path "", "Autosave Render"=FALSE, "Hide Labels"=FALSE, "Normal Render Path"=path "", "Overwrite"=FALSE} ("Configuration Data")
            # "Read Configuration Data from File"
            n490 = Unbundle By Name(w1272) -> ("Config"=w1271:refnum<class "Configuration.lvclass">)
            n491 = call <userlib>:"Read Configuration.vi"("INI Fomatted Cluster Type"=w1267, "error in (no error)"=w1269, "Configuration in"=w1271) -> ("error out"=w1265:errorcluster, "Configuration"=w1268:variant, "Configuration out"=w1270:refnum<class "Configuration.lvclass">)  [unwired: 6 in]
            n492 = Variant To Data(error in=w1265, type=w1267, Variant=w1268) -> (data=w1266:T11, error out=w1264:errorcluster)
            n493 = Unbundle(w1266) -> ("Inkscape Path"=w1263:path, "Background Path"=w1261:path, "Autosave Render Path"=w1260:path, "Autosave Render"=w1259:bool)  [unwired: 3 out]
            n494 = Bundle By Name(cluster=w1272, "Config"=w1270, "Inkscape File (.svg)"=w1263, "Background Image"=w1261, "Autosave Path"=w1260, "Autosave?"=w1259) -> (w1273:T20)
            n495 = call <vilib>:"Add State(s) to Queue__jki_lib_state_machine.vi"("State(s) in Front (\"\")"="UI: Status >> Configuration Read\nUI: Background Path\nUI: Inkscape Path\nUI: Autosave Render Path", "State(s) in (\"\")"=w1275) -> ("States Out"=w1276:string)  [unwired: 13 in]
          }
          frame "Configuration: Initialize" {
            # "Initialize Configuration Class with Path to File"
            n496 = Unbundle By Name(w1284) -> ("Config"=w1283:refnum<class "Configuration.lvclass">)
            n497 = call "Base INI Folder Path.vi"() -> ("Base Path"=w1278:path)  [unwired: 11 in]
            n498 = call <userlib>:"Write Path.vi"("error in (no error)"=w1280, "Filename [Configuration.ini]"="Config.ini" ("File (Configuration.ini)"), "Path"=w1278, "Configuration in"=w1283) -> ("error out"=w1281:errorcluster, "Configuration out"=w1282:refnum<class "Configuration.lvclass">)  [unwired: 6 in]
            n499 = Bundle By Name(cluster=w1284, "Config"=w1282) -> (w1285:T20)
            n500 = call <vilib>:"Add State(s) to Queue__jki_lib_state_machine.vi"("State(s) in Front (\"\")"="UI: Status >> Configuration Initialized" ("State(s) in Front (\"\")"), "State(s) in (\"\")"=w1287) -> ("States Out"=w1288:string)  [unwired: 13 in]
          }
          frame "---------- Driver ----------" {
            # "Template Separator\n(You can make a copy of, or modify, this frame)"
            n501 = call <vilib>:"Add State(s) to Queue__jki_lib_state_machine.vi"("State(s) in (\"\")"=w1290) -> ("States Out"=w1292:string)  [unwired: 14 in]
          }
          frame "Driver: Init Manager" {
            # "Template Separator\n(You can make a copy of, or modify, this frame)"
            n502 = Unbundle By Name(w1295) -> ("AFM_Driver_Manager"=w1300:refnum<class "AFM_Driver_Manager.lvclass">)
            n503 = call "AFM_Driver_Manager.Initialize.vi"("error in (no error)"=w1296, "AFM_Driver_Manager in"=w1300) -> ("error out"=w1297:errorcluster, "AFM_Driver_Manager out"=w1298:refnum<class "AFM_Driver_Manager.lvclass">)  [unwired: 8 in]
            n504 = Bundle By Name(cluster=w1295, "AFM_Driver_Manager"=w1298) -> (w1299:T20)
            n505 = call <vilib>:"Add State(s) to Queue__jki_lib_state_machine.vi"("State(s) in Front (\"\")"="UI: Status >> AFM Driver Manager Initialized" ("State(s) in Front (\"\")"), "State(s) in (\"\")"=w1302) -> ("States Out"=w1303:string)  [unwired: 13 in]
          }
          frame "Driver: Init Drivers" {
            # "Initialized an AFM_Driver_Manager Class using paths to the drivers.\n(All drivers will be started.)"
            n506 = Unbundle By Name(w1306) -> ("root path"=w1305:path)
            n507 = Unbundle By Name(w1306) -> ("AFM_Driver_Manager"=w1307:refnum<class "AFM_Driver_Manager.lvclass">)
            n508 = Build Path(base path=w1305, name or relative path="AFMs\\Asylum_Driver\\Asylum_Driver.vi") -> (appended path=w1311:path)
            n509 = Build Array(w1311) -> (w1310:path[])
            n510 = call "AFM_Driver_Manager.InitializeDrivers.vi"("error in (no error)"=w1314, "Paths"=w1310, "AFM_Driver_Manager in"=w1307) -> ("error out"=w1315:errorcluster, "AFM_Driver_Manager out"=w1312:refnum<class "AFM_Driver_Manager.lvclass">)  [unwired: 7 in]
            n511 = Bundle By Name(cluster=w1306, "AFM_Driver_Manager"=w1312) -> (w1313:T20)
            n512 = call <vilib>:"Add State(s) to Queue__jki_lib_state_machine.vi"("State(s) in Front (\"\")"="UI: Status >> AFM Driver Initialized" ("State(s) in Front (\"\")"), "State(s) in (\"\")"=w1316) -> ("States Out"=w1317:string)  [unwired: 13 in]
          }
          frame "Driver: Set Active" {
            # "Change the Active Driver. Call this state as Driver: Set Active >> # \n(where # is the panel to set active)"
            n513 = Decimal String To Number(string=w1320) -> (number=w1319:i32)  [unwired: 2 in, 1 out]
            n514 = Unbundle By Name(w1325) -> ("AFM_Driver_Manager"=w1324:refnum<class "AFM_Driver_Manager.lvclass">)
            n515 = call "AFM_Driver_Manager.SetActive.vi"("error in (no error)"=w1322, "Active Index"=w1319, "AFM_Driver_Manager in"=w1324) -> ("error out"=w1323:errorcluster, "AFM_Driver_Manager out"=w1326:refnum<class "AFM_Driver_Manager.lvclass">)  [unwired: 7 in]
            n516 = Bundle By Name(cluster=w1325, "AFM_Driver_Manager"=w1326) -> (w1327:T20)
            n517 = call <vilib>:"Add State(s) to Queue__jki_lib_state_machine.vi"("State(s) in Front (\"\")"="UI: Status >> Active Driver Selected" ("State(s) in Front (\"\")"), "State(s) in (\"\")"=w1328) -> ("States Out"=w1329:string)  [unwired: 13 in]
          }
          frame "Driver: Insert Into Subpanel" {
            # "Insert the Active Driver into the Subpanel provided\n(Active is by default panel 0)"
            n518 = Unbundle By Name(w1336) -> ("AFM_Driver_Manager"=w1338:refnum<class "AFM_Driver_Manager.lvclass">)
            n519 = control-ref of="AFM Settings"() -> (w1332:refnum<vi>)
            n520 = call "AFM_Driver_Manager.InsertActiveIntoSubpanel.vi"("error in (no error)"=w1333, "SubPnl Refnum"=w1332, "AFM_Driver_Manager in"=w1338) -> ("error out"=w1334:errorcluster, "AFM_Driver_Manager out"=w1335:refnum<class "AFM_Driver_Manager.lvclass">)  [unwired: 7 in]
            n521 = Bundle By Name(cluster=w1336, "AFM_Driver_Manager"=w1335) -> (w1337:T20)
            n522 = call <vilib>:"Add State(s) to Queue__jki_lib_state_machine.vi"("State(s) in Front (\"\")"="UI: Status >> AFM Driver inserted into subpanel" ("State(s) in Front (\"\")"), "State(s) in (\"\")"=w1339) -> ("States Out"=w1340:string)  [unwired: 13 in]
          }
          frame "Driver: Run Lithography" {
            # "Send a Command to the Driver to Run Lithography\n(You can make a copy of, or modify, this frame)"
            n523 = Unbundle By Name(w1344) -> ("AFM_Driver_Manager"=w1348:refnum<class "AFM_Driver_Manager.lvclass">)
            n524 = call "AFM_Driver_Manager.SendRun.vi"("error in (no error)"=w1346, "AFM_Driver_Manager in"=w1348) -> ("error out"=w1347:errorcluster, "AFM_Driver_Manager out"=w1343:refnum<class "AFM_Driver_Manager.lvclass">)  [unwired: 8 in]
            n525 = Bundle By Name(cluster=w1344, "AFM_Driver_Manager"=w1343) -> (w1345:T20)
            n526 = call <vilib>:"Add State(s) to Queue__jki_lib_state_machine.vi"("State(s) in Front (\"\")"="UI: Status >> Run Litho Msg Sent to Driver" ("State(s) in Front (\"\")"), "State(s) in (\"\")"=w1349) -> ("States Out"=w1350:string)  [unwired: 13 in]
          }
          frame "Driver: Litho Data" {
            # "Update the value of the lithography data in the driver\n(You can make a copy of, or modify, this frame)"
            n527 = Unbundle By Name(w1354) -> ("AFM_Driver_Manager"=w1358:refnum<class "AFM_Driver_Manager.lvclass">, "Lithography Data"=w1359:T27)
            n528 = call "AFM_Driver_Manager.SendLithography.vi"("error in (no error)"=w1351, "Lithography Data"=w1359, "AFM_Driver_Manager in"=w1358) -> ("error out"=w1352:errorcluster, "AFM_Driver_Manager out"=w1357:refnum<class "AFM_Driver_Manager.lvclass">)  [unwired: 7 in]
            n529 = Bundle By Name(cluster=w1354, "AFM_Driver_Manager"=w1357) -> (w1356:T20)
            n530 = call <vilib>:"Add State(s) to Queue__jki_lib_state_machine.vi"("State(s) in Front (\"\")"="UI: Status >> Lithography Data Sent to Driver" ("State(s) in Front (\"\")"), "State(s) in (\"\")"=w1360) -> ("States Out"=w1361:string)  [unwired: 13 in]
          }
          frame "Driver: Background Image" {
            # "Send the Background Image Path to the driver\n(You can make a copy of, or modify, this frame)"
            n531 = Unbundle By Name(w1364) -> ("AFM_Driver_Manager"=w1370:refnum<class "AFM_Driver_Manager.lvclass">, "Background Image"=w1363:path)
            n532 = call "AFM_Driver_Manager.SendBackgroundImage.vi"("error in (no error)"=w1368, "Path"=w1363, "AFM_Driver_Manager in"=w1370) -> ("error out"=w1369:errorcluster, "AFM_Driver_Manager out"=w1366:refnum<class "AFM_Driver_Manager.lvclass">)  [unwired: 7 in]
            n533 = Bundle By Name(cluster=w1364, "AFM_Driver_Manager"=w1366) -> (w1367:T20)
            n534 = call <vilib>:"Add State(s) to Queue__jki_lib_state_machine.vi"("State(s) in Front (\"\")"="UI: Status >> Background Image Sent to Driver" ("State(s) in Front (\"\")"), "State(s) in (\"\")"=w1371) -> ("States Out"=w1372:string)  [unwired: 13 in]
          }
          frame "Driver: Stop Manager" {
            # "Stops all drivers.\n(You can make a copy of, or modify, this frame)"
            n535 = Unbundle By Name(w1378) -> ("AFM_Driver_Manager"=w1377:refnum<class "AFM_Driver_Manager.lvclass">)
            n536 = call "AFM_Driver_Manager.Shutdown.vi"("error in (no error)"=w1375, "AFM_Driver_Manager in"=w1377) -> ("error out"=w1376:errorcluster)  [unwired: 9 in]
            n537 = call <vilib>:"Add State(s) to Queue__jki_lib_state_machine.vi"("State(s) in Front (\"\")"="UI: Status >> AFM Driver Manager Shut Down" ("State(s) in Front (\"\")"), "State(s) in (\"\")"=w1379) -> ("States Out"=w1380:string)  [unwired: 13 in]
          }
          frame "---------- Parser ----------" {
            # "Template Separator\n(You can make a copy of, or modify, this frame)"
            n538 = Unbundle By Name(w1382) -> ("ParseVectorFile"=w1381:refnum<class "ParseVectorFile.lvclass">)
            n539 = Bundle By Name(cluster=w1382, "ParseVectorFile"=w1381) -> (w1383:T20)
            n540 = call <vilib>:"Add State(s) to Queue__jki_lib_state_machine.vi"("State(s) in (\"\")"=w1385) -> ("States Out"=w1386:string)  [unwired: 14 in]
          }
          frame "Parser: Parse SVG" {
            # "New parser is about 1/2 the speed of old parser (~15 ms vs ~35 ms), but is better in almost every other aspect that actually counts"
            # "Parses an SVG file\n(You can make a copy of, or modify, this frame)"
            n541 = Unbundle By Name(w1415) -> ("Tooler"=w1411:refnum<class "Tool Data.lvclass">, "ParseVectorFile"=w1413:refnum<class "ParseVectorFile.lvclass">, "Inkscape File (.svg)"=w1414:path)
            n542 = call "ParseVectorFile.NewFileSynchronous.vi"("timeout in ms (-1)"=20000, "error in (no error)"=w1391, "Path"=w1414, "ParseVectorFile"=w1413) -> ("error out"=w1389:errorcluster, "ParsedData"=w1407:T34, "ParseVectorFile out"=w1397:refnum<class "ParseVectorFile.lvclass">)  [unwired: 5 in]
            n543 = Unbundle By Name(w1407) -> ("Paths"=w1406:refnum<class "Path.lvclass">[], "Rectangles"=w1405:refnum<class "Rectangle.lvclass">[], "Background"=w1390:refnum<class "SVGImage.lvclass">, "Dots"=w1404:refnum<class "Dot.lvclass">[])
            n544 = call-dynamic "Read Data.vi"("error in (no error)"=w1389, "Tool Data in"=w1411) -> ("error out"=w1388:errorcluster, "Data"=w1409:T35, "Tool Data out"=w1410:refnum<class "Tool Data.lvclass">)  [unwired: 7 in]
            n545 = property class="SVGImage.lvclass"(reference=w1390) -> ("Accessors:Height"=w1394:dbl, "Accessors:Width"=w1393:dbl)  [unwired: 1 in, 2 out]
            n546 = Bundle By Name(cluster=w1409, "Paths"=w1406, "Rectangles"=w1405, "SVGImage"=w1390, "Dots"=w1404) -> (w1408:T35)
            n547 = call-dynamic "Write Data.vi"("error in (no error)"=w1388, "Data"=w1408, "Tool Data in"=w1410) -> ("error out"=w1403:errorcluster, "Tool Data out"=w1398:refnum<class "Tool Data.lvclass">)  [unwired: 7 in]
            n548 = Bundle By Name(cluster=cluster{"Width":dbl, "Height":dbl} {"Width"=0.0, "Height"=0.0} ("Image Size In"), "Height"=w1394, "Width"=w1393) -> (w1392:cluster{"Width":dbl, "Height":dbl})
            n549 = call "Sort Funnels and Paths.vi"("error in (no error)"=w1403, "Tool Data in"=w1398) -> ("error out"=w1401:errorcluster, "Tool Data out"=w1402:refnum<class "Tool Data.lvclass">)  [unwired: 8 in]
            n550 = call "Set Inkscape Ratio.vi"("Image Size In"=w1392) -> ("Image Size Out"=w1417:cluster{"Width":dbl, "Height":dbl})
            n551 = call "Get IDs.vi"("error in (no error)"=w1401, "Tool Data in"=w1402) -> ("error out"=w1400:errorcluster, "IDs"=w1399:T24)  [unwired: 7 in, 1 out]
            n552 = Bundle By Name(cluster=w1415, "Tooler"=w1398, "ParseVectorFile"=w1397, "IDs"=w1399) -> (w1416:T20)
            n553 = global write "Global Variables.vi" "Size"(w1417) -> ()
            n554 = call <vilib>:"Add State(s) to Queue__jki_lib_state_machine.vi"("State(s) in Front (\"\")"="UI: Status >> File parsed.\nMCLB: Generate Names" ("State(s) in Front (\"\")"), "State(s) in (\"\")"=w1419) -> ("States Out"=w1420:string)  [unwired: 13 in]
          }
          frame "Parser: Stop" {
            # "Template Separator\n(You can make a copy of, or modify, this frame)"
            n555 = Unbundle By Name(w1428) -> ("ParseVectorFile"=w1425:refnum<class "ParseVectorFile.lvclass">)
            n556 = call <vilib>:"Stop.vi"("error in (no error)"=w1423, "SMO"=w1425) -> ("error out"=w1426:errorcluster, "SMO out"=w1427:refnum<class "ParseVectorFile.lvclass">)  [unwired: 8 in]
            n557 = call <vilib>:"Destroy.vi"("error in (no error)"=w1426, "SMO"=w1427) -> ("error out"=w1424:errorcluster)  [unwired: 9 in]
            n558 = Bundle By Name(cluster=w1428, "ParseVectorFile"=refnum<class "ParseVectorFile.lvclass"> refnum) -> (w1429:T20)
            n559 = call <vilib>:"Add State(s) to Queue__jki_lib_state_machine.vi"("State(s) in Front (\"\")"="UI: Status >> Parser Stopped" ("State(s) in Front (\"\")"), "State(s) in (\"\")"=w1431) -> ("States Out"=w1432:string)  [unwired: 13 in]
          }
          frame "Parser: Start" {
            # "Template Separator\n(You can make a copy of, or modify, this frame)"
            n560 = Unbundle By Name(w1440) -> ("ParseVectorFile"=w1439:refnum<class "ParseVectorFile.lvclass">)
            n561 = call <vilib>:"Create.vi"("error in (no error)"=w1434, "SMO"=w1439) -> ("error out"=w1436:errorcluster, "SMO out"=w1438:refnum<class "ParseVectorFile.lvclass">)  [unwired: 7 in, 1 out]
            n562 = call <vilib>:"Start.vi"("error in (no error)"=w1436, "SMO"=w1438) -> ("error out"=w1435:errorcluster, "SMO out"=w1437:refnum<class "ParseVectorFile.lvclass">)  [unwired: 8 in]
            n563 = Bundle By Name(cluster=w1440, "ParseVectorFile"=w1437) -> (w1441:T20)
            n564 = call <vilib>:"Add State(s) to Queue__jki_lib_state_machine.vi"("State(s) in Front (\"\")"="UI: Status >> Parser started." ("State(s) in Front (\"\")"), "State(s) in (\"\")"=w1443) -> ("States Out"=w1444:string)  [unwired: 13 in]
          }
          frame "---------- Database ----------" {
            # "Template Separator\n(You can make a copy of, or modify, this frame)"
            n565 = Unbundle By Name(w1446) -> ("Database"=w1445:refnum<class "Setting Database.lvclass">)
            n566 = Bundle By Name(cluster=w1446, "Database"=w1445) -> (w1447:T20)
            n567 = call <vilib>:"Add State(s) to Queue__jki_lib_state_machine.vi"("State(s) in (\"\")"=w1449) -> ("States Out"=w1450:string)  [unwired: 14 in]
          }
          frame "Database: Update Enable" {
            # "Template Separator\n(You can make a copy of, or modify, this frame)"
            n568 = Unbundle By Name(w1457) -> ("Database"=w1456:refnum<class "Setting Database.lvclass">)
            n569 = call "Setting Database.ChangeObjectEnable.vi"("error in (no error)"=w1453, "ChangeObjectEnable"=w1452, "Setting Database"=w1456) -> ("error out"=w1454:errorcluster, "Setting Database out"=w1455:refnum<class "Setting Database.lvclass">)  [unwired: 7 in]
            n570 = Bundle By Name(cluster=w1457, "Database"=w1455) -> (w1458:T20)
            n571 = call <vilib>:"Add State(s) to Queue__jki_lib_state_machine.vi"("State(s) in (\"\")"=w1460) -> ("States Out"=w1461:string)  [unwired: 14 in]
          }
          frame "Database: Set Active" {
            # "Template Separator\n(You can make a copy of, or modify, this frame)"
            n572 = call "Name To Type.vi"("Name"=w1462) -> ("Type"=w1464:string)  [unwired: 4 in]
            n573 = call "Name To Index.vi"("Name"=w1462) -> ("Index"=w1463:i32)  [unwired: 4 in]
            n574 = Unbundle By Name(w1470) -> ("Database"=w1469:refnum<class "Setting Database.lvclass">)
            n575 = case shown="\"d\"" w1464 {
              tunnel: w1469 -> [w1479 w1481 w1486 w1491 w1496 w1500]
              tunnel: [w1478 w1480 w1485 w1489 w1494 w1499] -> w1468
              tunnel: w1467 -> [w1475 w1480 w1484 w1488 w1493 w1498]
              tunnel: [w1479 w1481 w1483 w1490 w1495 w1501] -> w1466
              tunnel: w1463 -> [_ _ w1482 w1487 w1492 w1497]
              frame Default {
                n576 = call <vilib>:"Error Cluster From Error Code.vi"("error in (no error)"=w1475, "error message (\"\")"="Unknown Object Type. Cannot Set Active In Database" ("error message (\"\")"), "error code (0)"=1) -> ("error out"=w1478:errorcluster)  [unwired: 6 in]
              }
              frame "" {
                # "There are no objects to set as active\n\nTemp fix for issue \\#78:\nhttps://github.com/levylabpitt/AFM-Lithography/issues/78"
              }
              frame "p" {
                n577 = call "Setting Database.SetActivePath.vi"("error in (no error)"=w1484, "SetActivePath"=w1482, "Setting Database"=w1486) -> ("error out"=w1485:errorcluster, "Setting Database out"=w1483:refnum<class "Setting Database.lvclass">)  [unwired: 7 in]
              }
              frame "r" {
                n578 = call "Setting Database.SetActiveRectangle.vi"("error in (no error)"=w1488, "SetActiveRectangle"=w1487, "Setting Database"=w1491) -> ("error out"=w1489:errorcluster, "Setting Database out"=w1490:refnum<class "Setting Database.lvclass">)  [unwired: 7 in]
              }
              frame "f" {
                n579 = call "Setting Database.SetActiveFunnel.vi"("error in (no error)"=w1493, "SetActiveFunnel"=w1492, "Setting Database"=w1496) -> ("error out"=w1494:errorcluster, "Setting Database out"=w1495:refnum<class "Setting Database.lvclass">)  [unwired: 7 in]
              }
              frame "d" {
                # "Need to send the data event here"
                n580 = call "Setting Database.SetActiveDot.vi"("error in (no error)"=w1498, "SetActiveDot"=w1497, "Setting Database"=w1500) -> ("error out"=w1499:errorcluster, "Setting Database out"=w1501:refnum<class "Setting Database.lvclass">)  [unwired: 7 in]
              }
            }
            n581 = Bundle By Name(cluster=w1470, "Database"=w1466) -> (w1471:T20)
            n582 = call <vilib>:"Add State(s) to Queue__jki_lib_state_machine.vi"("State(s) in Front (\"\")"="UI: Status >> Database: Active Object Set" ("State(s) in Front (\"\")"), "State(s) in (\"\")"=w1473) -> ("States Out"=w1474:string)  [unwired: 13 in]
          }
          frame "Database: Refresh" {
            # "This can be updated to have IDs, which will allow for more control over keeping settings"
            # "Handle UI changes to account for the fact that the active value is once again zero. I am treating it like a click (generating a UI Event with the signalling property) because I want to go through the logic as if it was identical to a user selecting a different value."
            # "Template Separator\n(You can make a copy of, or modify, this frame)"
            n583 = Unbundle By Name(w1517) -> ("Database"=w1516:refnum<class "Setting Database.lvclass">, "IDs.paths"=w1505:string[], "IDs.funnels"=w1504:string[], "IDs.rects"=w1503:string[], "IDs.dots"=w1502:string[])
            n584 = Bundle By Name(cluster=T12 {"Paths"=[], "Rectangles"=[], "Funnels"=[], "Dots"=[]} ("Initialize"), "Paths"=w1505, "Funnels"=w1504, "Rectangles"=w1503, "Dots"=w1502) -> (w1513:T12)
            n585 = call "Setting Database.Refresh.vi"("error in (no error)"=w1508, "Initialize"=w1513, "Setting Database"=w1516) -> ("error out"=w1510:errorcluster, "Setting Database out"=w1515:refnum<class "Setting Database.lvclass">)  [unwired: 7 in]
            n586 = control-ref of="Patterns"() -> (w1512:refnum<vi>)
            n587 = property class="LstBox (strict)"(reference=w1512, error in=w1510, "Val(Sgnl)"=0 ("Value")) -> (error out=w1507:errorcluster)  [unwired: 1 out]
            n588 = Bundle By Name(cluster=w1517, "Database"=w1515) -> (w1518:T20)
            n589 = Merge Errors(w1507) -> (w1506:errorcluster)
            n590 = call <vilib>:"Add State(s) to Queue__jki_lib_state_machine.vi"("State(s) in Front (\"\")"="UI: Status >> Database Refresh Msg Sent" ("State(s) in Front (\"\")"), "State(s) in (\"\")"=w1520) -> ("States Out"=w1521:string)  [unwired: 13 in]
          }
          frame "Database: Refresh Sync" {
            # "#issue\nThis might be the cause of the odd timing in the order data VI?"
            # "Template Separator\n(You can make a copy of, or modify, this frame)"
            n591 = Unbundle By Name(w1556) -> ("Database"=w1552:refnum<class "Setting Database.lvclass">, "IDs.paths"=w1540:string[], "IDs.funnels"=w1539:string[], "IDs.rects"=w1538:string[], "IDs.dots"=w1537:string[], "Tooler"=w1534:refnum<class "Tool Data.lvclass">)
            n592 = control-ref of="Patterns"() -> (w1554:refnum<vi>)
            n593 = property class="LstBox (strict)"(reference=w1554, error in=w1543, "Value"=0) -> (error out=w1542:errorcluster)  [unwired: 1 out]
            n594 = Bundle By Name(cluster=T12 {"Paths"=[], "Rectangles"=[], "Funnels"=[], "Dots"=[]} ("Initialize"), "Paths"=w1540, "Funnels"=w1539, "Rectangles"=w1538, "Dots"=w1537) -> (w1550:T12)
            n595 = Merge Errors(w1542) -> (w1541:errorcluster)
            n596 = call <userlib>:"Tick Count (ms)__ogtk.vi"("error in (no error)"=w1541) -> ("error out"=w1547:errorcluster, "millisecond timer value"=w1545:u32)  [unwired: 9 in]
            n597 = call "Setting Database.Refresh.Synchronous.vi"("Timeout"=-1, "error in (no error)"=w1547, "Initialize"=w1550, "Setting Database in"=w1552) -> ("error out"=w1525:errorcluster, "Response"=w1531:T21, "Setting Database out"=w1551:refnum<class "Setting Database.lvclass">)  [unwired: 5 in]
            n598 = Unbundle By Name(w1531) -> ("Paths"=w1530:T14, "Rectangles"=w1529:T15, "Funnels"=w1528:T16, "Dots"=w1527:T17)
            n599 = call-dynamic "Read Settings.vi"("error in (no error)"=w1525, "Tool Data in"=w1534) -> ("error out"=w1526:errorcluster, "Settings"=w1533:T21, "Tool Data out"=w1535:refnum<class "Tool Data.lvclass">)  [unwired: 7 in]
            n600 = Bundle By Name(cluster=w1533, "Paths"=w1530, "Rectangles"=w1529, "Funnels"=w1528, "Dots"=w1527) -> (w1532:T21)
            n601 = call <userlib>:"Tick Count (ms)__ogtk.vi"("error in (no error)"=w1525) -> ("error out"=w1524:errorcluster, "millisecond timer value"=w1546:u32)  [unwired: 9 in]
            n602 = call-dynamic "Write Settings.vi"("error in (no error)"=w1526, "Settings"=w1532, "Tool Data in"=w1535) -> ("error out"=w1523:errorcluster, "Tool Data out"=w1536:refnum<class "Tool Data.lvclass">)  [unwired: 7 in]
            n603 = Subtract(x=w1546, y=w1545) -> ()  [unwired: 1 out]
            n604 = Bundle By Name(cluster=w1556, "Database"=w1551, "Tooler"=w1536) -> (w1557:T20)
            n605 = Merge Errors(w1523, w1524) -> (w1522:errorcluster)
            n606 = call <vilib>:"Add State(s) to Queue__jki_lib_state_machine.vi"("State(s) in Front (\"\")"="UI: Status >> Database Refreshed (Sync)" ("State(s) in Front (\"\")"), "State(s) in (\"\")"=w1559, "State(s) at Back (\"\")"="UI: Status >> New Active Object Selected\nMCLB: Symbols\nUI: Update Subpanel\nLitho: Order Data\nDriver: Litho Data" ("State(s) at Back (\"\")")) -> ("States Out"=w1560:string)  [unwired: 12 in]
          }
          frame "Database: Start" {
            # "Shared resource"
            # "This needs to be called before the Path Edit is started, otherwise path edit wont be able to find the shared resource"
            # "Template Separator\n(You can make a copy of, or modify, this frame)"
            n607 = Unbundle By Name(w1571) -> ("Database"=w1566:refnum<class "Setting Database.lvclass">)
            n608 = call "Setting Database Name.vi"("error in (no error)"=w1562) -> ("error out"=w1563:errorcluster, "Name"=w1568:string)  [unwired: 9 in]
            n609 = call <vilib>:"Create.vi"("Shared Resource (F)"=TRUE, "error in (no error)"=w1563, "Subsystem Name (optional)"=w1568, "SMO"=w1566) -> ("error out"=w1567:errorcluster, "SMO out"=w1570:refnum<class "Setting Database.lvclass">)  [unwired: 5 in, 1 out]
            n610 = call <vilib>:"Start.vi"("error in (no error)"=w1567, "SMO"=w1570) -> ("error out"=w1564:errorcluster, "SMO out"=w1565:refnum<class "Setting Database.lvclass">)  [unwired: 8 in]
            n611 = Bundle By Name(cluster=w1571, "Database"=w1565) -> (w1572:T20)
            n612 = call <vilib>:"Add State(s) to Queue__jki_lib_state_machine.vi"("State(s) in Front (\"\")"="UI: Status >> Settings Database Started" ("State(s) in Front (\"\")"), "State(s) in (\"\")"=w1574) -> ("States Out"=w1575:string)  [unwired: 13 in]
          }
          frame "Database: Stop" {
            # "Only call this on shutdown, otherwise it might cause problems with shared resource."
            # "Template Separator\n(You can make a copy of, or modify, this frame)"
            n613 = Unbundle By Name(w1583) -> ("Database"=w1581:refnum<class "Setting Database.lvclass">)
            n614 = call <vilib>:"Stop.vi"("error in (no error)"=w1577, "SMO"=w1581) -> ("error out"=w1579:errorcluster, "SMO out"=w1580:refnum<class "Setting Database.lvclass">)  [unwired: 8 in]
            n615 = call <vilib>:"Destroy.vi"("error in (no error)"=w1579, "SMO"=w1580) -> ("error out"=w1578:errorcluster)  [unwired: 9 in]
            n616 = Bundle By Name(cluster=w1583, "Database"=refnum<class "Setting Database.lvclass"> refnum) -> (w1584:T20)
            n617 = call <vilib>:"Add State(s) to Queue__jki_lib_state_machine.vi"("State(s) in Front (\"\")"="UI: Status >> Settings Database Stopped" ("State(s) in Front (\"\")"), "State(s) in (\"\")"=w1586) -> ("States Out"=w1587:string)  [unwired: 13 in]
          }
          frame "---------- Tooler ----------" {
            # "Template Separator\n(You can make a copy of, or modify, this frame)"
            n618 = Unbundle By Name(w1590) -> ("Tooler"=w1588:refnum<class "Tool Data.lvclass">)
            n619 = Bundle By Name(cluster=w1590, "Tooler"=w1588) -> (w1591:T20)
            n620 = call <vilib>:"Add State(s) to Queue__jki_lib_state_machine.vi"("State(s) in (\"\")"=w1593) -> ("States Out"=w1594:string)  [unwired: 14 in]
          }
          frame "Tooler: Stop" {
            # "Template Separator\n(You can make a copy of, or modify, this frame)"
            n621 = Unbundle By Name(w1601) -> ("Tooler"=w1600:refnum<class "Tool Data.lvclass">)
            n622 = call <vilib>:"Stop.vi"("error in (no error)"=w1595, "SMO"=w1600) -> ("error out"=w1597:errorcluster, "SMO out"=w1599:refnum<class "Tool Data.lvclass">)  [unwired: 8 in]
            n623 = call <vilib>:"Destroy.vi"("error in (no error)"=w1597, "SMO"=w1599) -> ("error out"=w1596:errorcluster)  [unwired: 9 in]
            n624 = Bundle By Name(cluster=w1601, "Tooler"=refnum<class "Tool Data.lvclass"> refnum) -> (w1602:T20)
            n625 = call <vilib>:"Add State(s) to Queue__jki_lib_state_machine.vi"("State(s) in (\"\")"=w1604) -> ("States Out"=w1605:string)  [unwired: 14 in]
          }
          frame "Tooler: Start" {
            # "Template Separator\n(You can make a copy of, or modify, this frame)"
            n626 = Unbundle By Name(w1612) -> ("Tooler"=w1609:refnum<class "Tool Data.lvclass">)
            n627 = call <vilib>:"Create.vi"("error in (no error)"=w1606, "SMO"=w1609) -> ("error out"=w1611:errorcluster, "SMO out"=w1610:refnum<class "Tool Data.lvclass">)  [unwired: 7 in, 1 out]
            n628 = call <vilib>:"Start.vi"("error in (no error)"=w1611, "SMO"=w1610) -> ("error out"=w1607:errorcluster, "SMO out"=w1608:refnum<class "Tool Data.lvclass">)  [unwired: 8 in]
            n629 = Bundle By Name(cluster=w1612, "Tooler"=w1608) -> (w1613:T20)
            n630 = call <vilib>:"Add State(s) to Queue__jki_lib_state_machine.vi"("State(s) in (\"\")"=w1615) -> ("States Out"=w1616:string)  [unwired: 14 in]
          }
          frame "Tooler: Objects" {
            # "Template Separator\n(You can make a copy of, or modify, this frame)"
            n631 = Unbundle By Name(w1642) -> ("Tooler"=w1640:refnum<class "Tool Data.lvclass">)
            n632 = call-dynamic "Read Data.vi"("error in (no error)"=w1631, "Tool Data in"=w1640) -> ("error out"=w1632:errorcluster, "Data"=w1634:T35, "Tool Data out"=w1639:refnum<class "Tool Data.lvclass">)  [unwired: 7 in]
            n633 = call-dynamic "Read Settings.vi"("error in (no error)"=w1632, "Tool Data in"=w1639) -> ("error out"=w1633:errorcluster, "Settings"=w1635:T21, "Tool Data out"=w1638:refnum<class "Tool Data.lvclass">)  [unwired: 7 in]
            n634 = Bundle By Name(cluster=T13 {"Settings"={"Paths"=[], "Rectangles"=[], "Funnels"=[], "Dots"=[]}, "Data"={"Paths"=[], "Rectangles"=[], "SVGImage"=refnum, "Dots"=[], "Funnels"=[]}} ("Update Objects"), "Settings"=w1635, "Data"=w1634) -> (w1636:T13)
            n635 = call-dynamic "Tool Data.ToolObjectsSynchronous.vi"("Timeout"=20000, "error in (no error)"=w1633, "Update Objects"=w1636, "Tool Data in"=w1638) -> ("error out"=w1626:errorcluster, "Object Updated"=w1624:T36, "Tool Data out"=w1628:refnum<class "Tool Data.lvclass">)  [unwired: 5 in]
            n636 = call-dynamic "Write Tooled.vi"("error in (no error)"=w1626, "Tooled"=w1624, "Tool Data in"=w1628) -> ("error out"=w1625:errorcluster, "Tool Data out"=w1627:refnum<class "Tool Data.lvclass">)  [unwired: 7 in]
            n637 = call-dynamic "Generate Lithography Data.vi"("error in (no error)"=w1625, "Tool Data in"=w1627) -> ("error out"=w1629:errorcluster, "Lithography Data"=w1617:T27, "Tool Data out"=w1630:refnum<class "Tool Data.lvclass">)  [unwired: 7 in]
            n638 = call "Estimated Time Required.vi"("Lithography Data"=w1617) -> ("Estimated Time Required"=w1622:timestamp)
            n639 = for {
              tunnel: w1617 -> [w1648] mode=indexing
              tunnel: [w1647] -> w1618 mode=indexing
              n640 = Unbundle By Name(w1648) -> ("Name"=w1647:string)
            }
            n641 = Format Date/Time String(time format string (%c)="%H:%M:%S", seconds (now)=w1622) -> (date/time string=w1621:string)  [unwired: 1 in]
            n642 = Bundle By Name(cluster=w1642, "Tooler"=w1630, "Lithography Data"=w1617, "Drag and Drop.Working"=w1618) -> (w1643:T20)
            n643 = call <vilib>:"Build State String with Arguments__JKI_lib_State_Machine.vi"("Arguments (\"\")"=w1621, "State"="UI: Update Time") -> ("State with Arguments"=w1619:string)  [unwired: 4 in]
            n644 = call <vilib>:"Add State(s) to Queue__jki_lib_state_machine.vi"("State(s) in Front (\"\")"=w1619, "State(s) in (\"\")"=w1645) -> ("States Out"=w1646:string)  [unwired: 13 in]
          }
        }
        n645 = call <userlib>:"Tick Count (ms)__ogtk.vi"("error in (no error)"=w27) -> ("error out"=w24:errorcluster, "millisecond timer value"=w22:u32)  [unwired: 9 in]
        n646 = Subtract(x=w22, y=w21) -> (x-y=w20:u32)
      }
    }
    frame Enabled {
    }
  }
  n647 = for {
    tunnel: w4 -> [w1652] mode=indexing
    tunnel: w3 -> [w1653] mode=indexing
    tunnel: [w1649] -> w1 mode=indexing
    n648 = Number To Decimal String(number=w1653) -> (decimal integer string=w1650:string)  [unwired: 1 in]
    n649 = Concatenate Strings(w1652, "     " ("string"), w1650) -> (w1649:string)
  }
  n650 = control-ref of="Listbox"() -> (w2:refnum<vi>)
  n651 = property class="LstBox (strict)"(reference=w2, "Item Names"=w1) -> ()  [unwired: 1 in, 2 out]
